vi "BuildRelease.vi"() -> ()   [LabVIEW 2020]
uses:
  <vilib>/Utility/traverseref.llb/TRef TravTarget.ctl
  <vilib>/Utility/traverseref.llb/VI Scripting - Traverse.lvlib
panel:
  out "error out":errorcluster
  out "Tab":enum32{"Start", "Building"}(tab)
  in  "Package Build":i32
  in  "AutoInstallAfterBuild":bool
  in  "DeleteRelease":bool
  in  "Output Folder":path=path "C:/OpenGDS" caption="Build folder: C:\\OpenGDS\\1.2.87(Master)"
  in  "LV_Versions":cluster{"LvVersion":string, "Check":bool}[](array[cluster]) caption="LV versions to compile the release for"
  in  "Build":bool
  out "Branch Name":string
  in  "New Version Number":string
  out "Current Version Number":string
  out "Progress":u8(slide) scale=0.0..100.0
  out "Progress":string
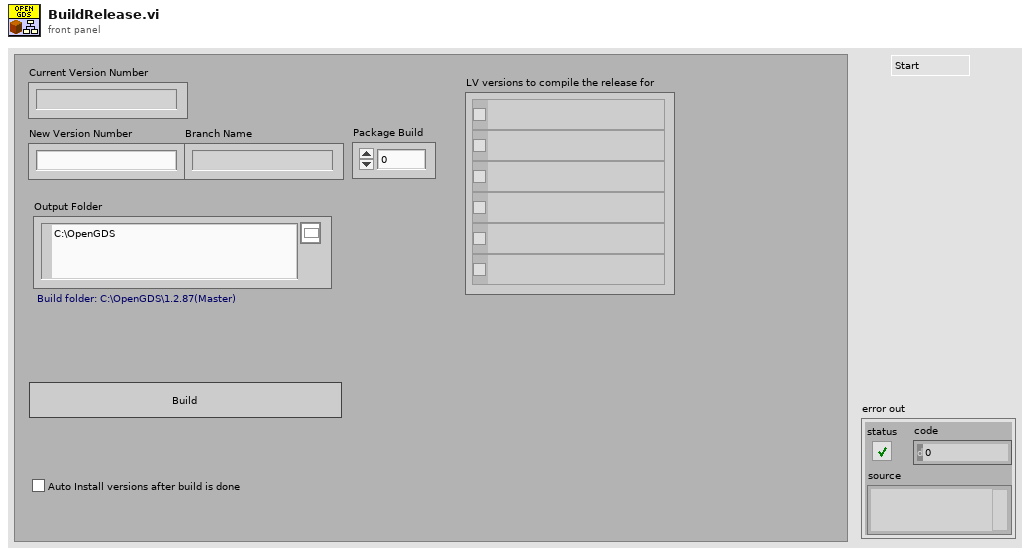
[diagram p1: front panel]
types:
  T1 = cluster{"LvVersion":path[], "BuildPath":path, "SourceFiles":path[], "LvVersion":string[], "SpecFile":path, "IniFiles":path[], "InstallerCopy":path, "VersionName":string, "InstallerFile":path, "ReadMeFile":path, "VIP-File":path, "LogFolder":path, "ZipFilesCreated":path[]}
  T2 = enum32{"invalid OS target", "Mac OS", "Windows 3.1", "Windows 95/NT", "Solaris 1", "Solaris 2", "HP-UX", "PowerMAX", "Linux", "Irix", "Rhapsody", "BeOS", "AIX", "OSF1", "VxWorks", "PharLap", "Carbon", "RTX", "Windows x64", "Linux x64"}
  T3 = enum8{"Enabled", "Disabled", "Disabled and Grayed Out"}
  T4 = typedef "TRef TravTarget.ctl" = enum16{"FP", "BD", "Other"}
  T5 = enum32{"invalid OS target", "Mac OS", "Windows 3.1", "Windows 95/NT", "Solaris 1", "Solaris 2", "HP-UX", "PowerMAX", "Linux", "Irix", "Rhapsody", "BeOS", "AIX", "OSF1", "VxWorks", "PharLap", "Carbon", "RTX", "Windows x64", "Linux x64", "Mac OS X x64"}
  T6 = enum32{"not a typedef", "typedef", "strict typedef", "class private data"}
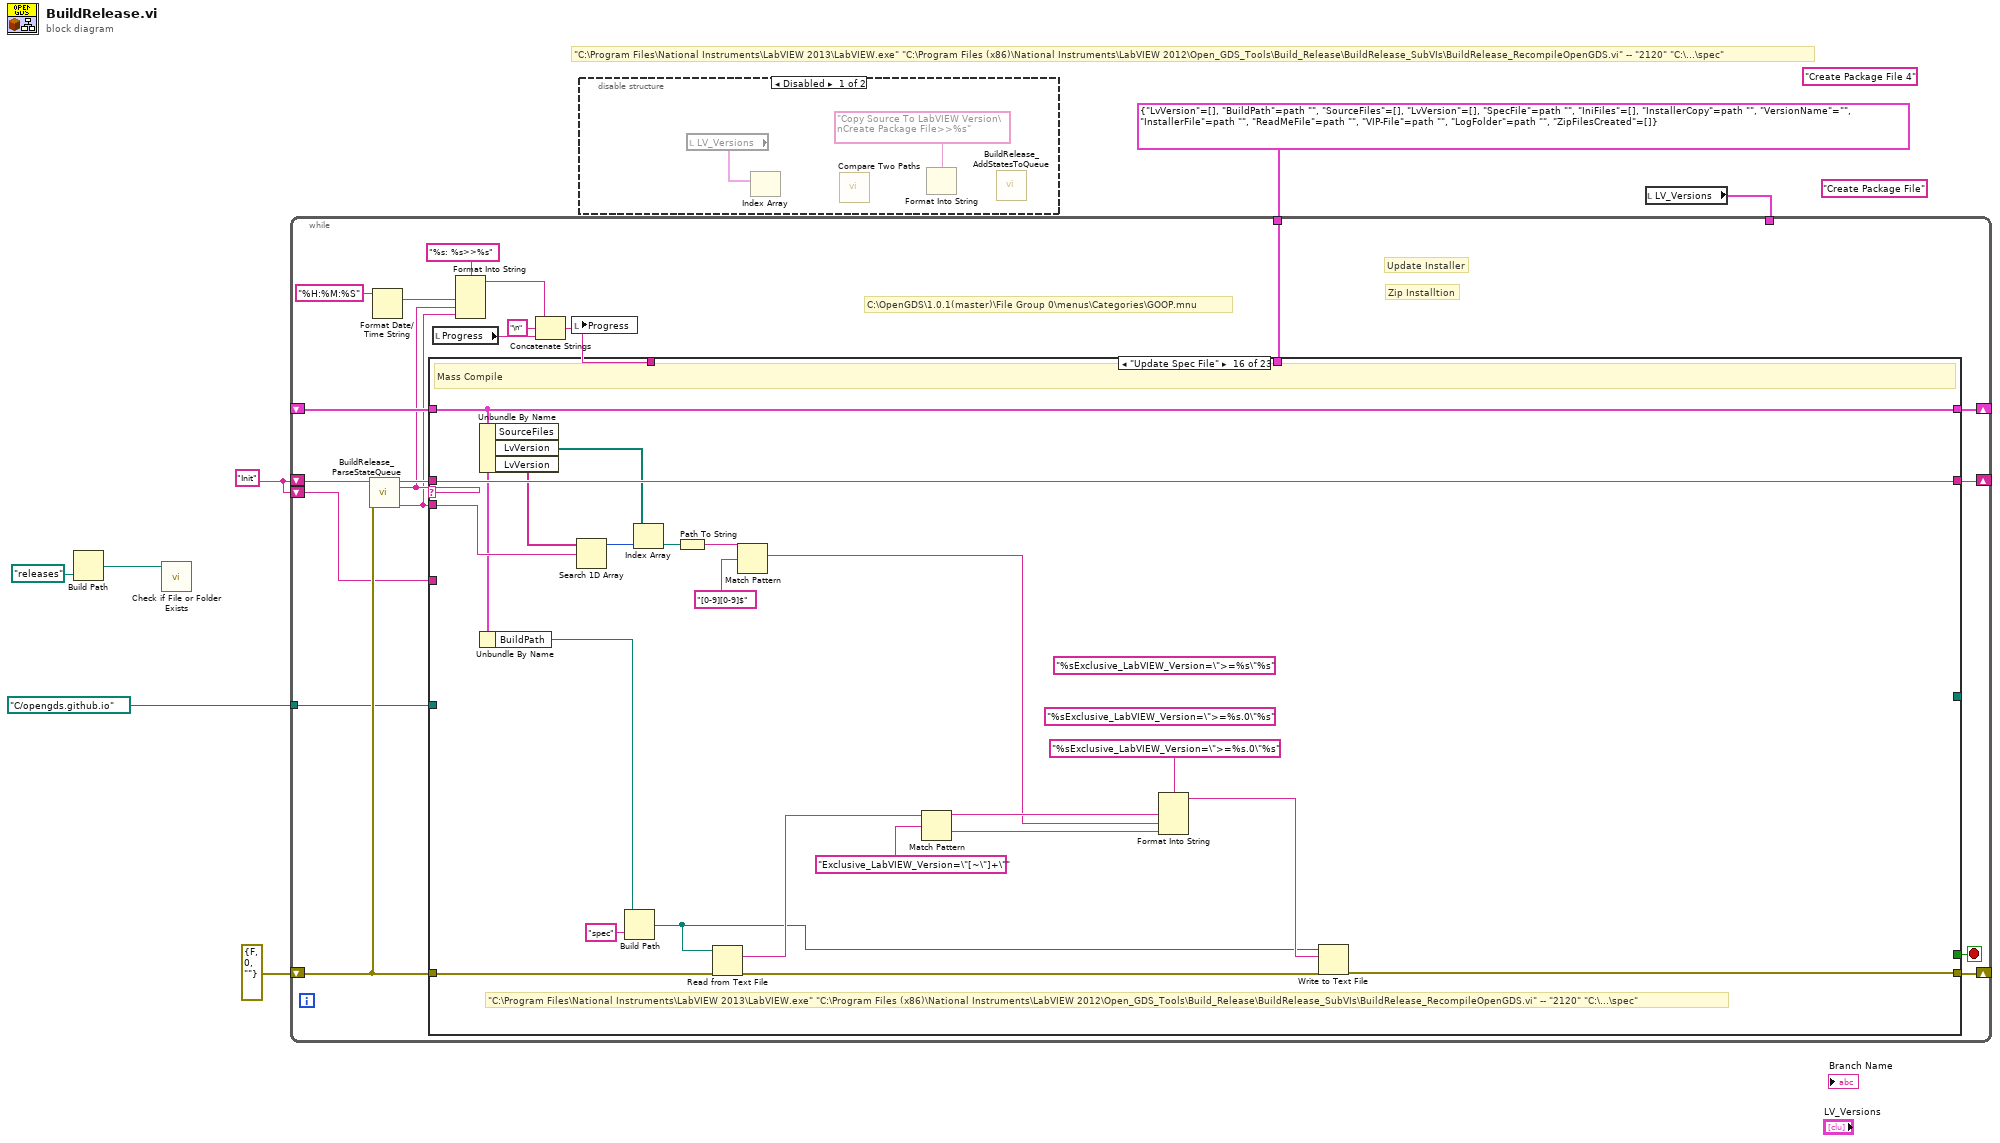
[diagram p0: block diagram]
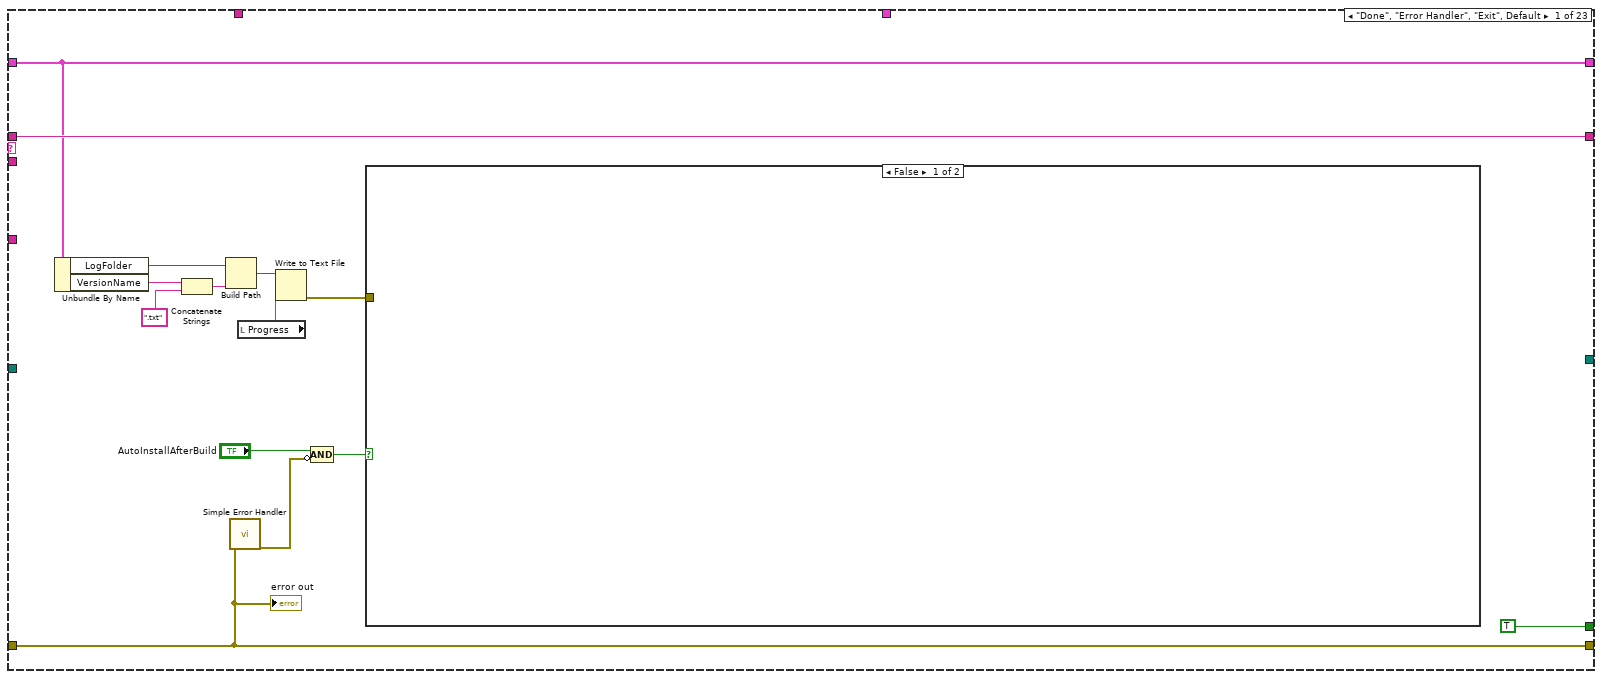
[diagram p3: hidden frame]
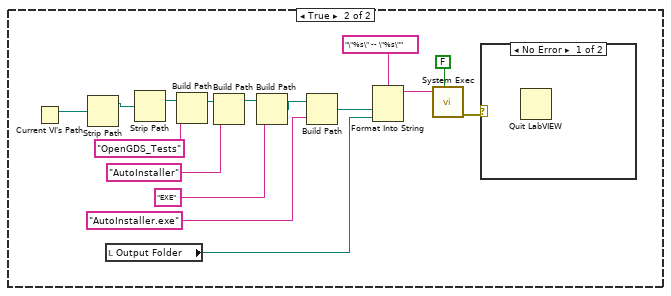
[diagram p4: hidden frame]
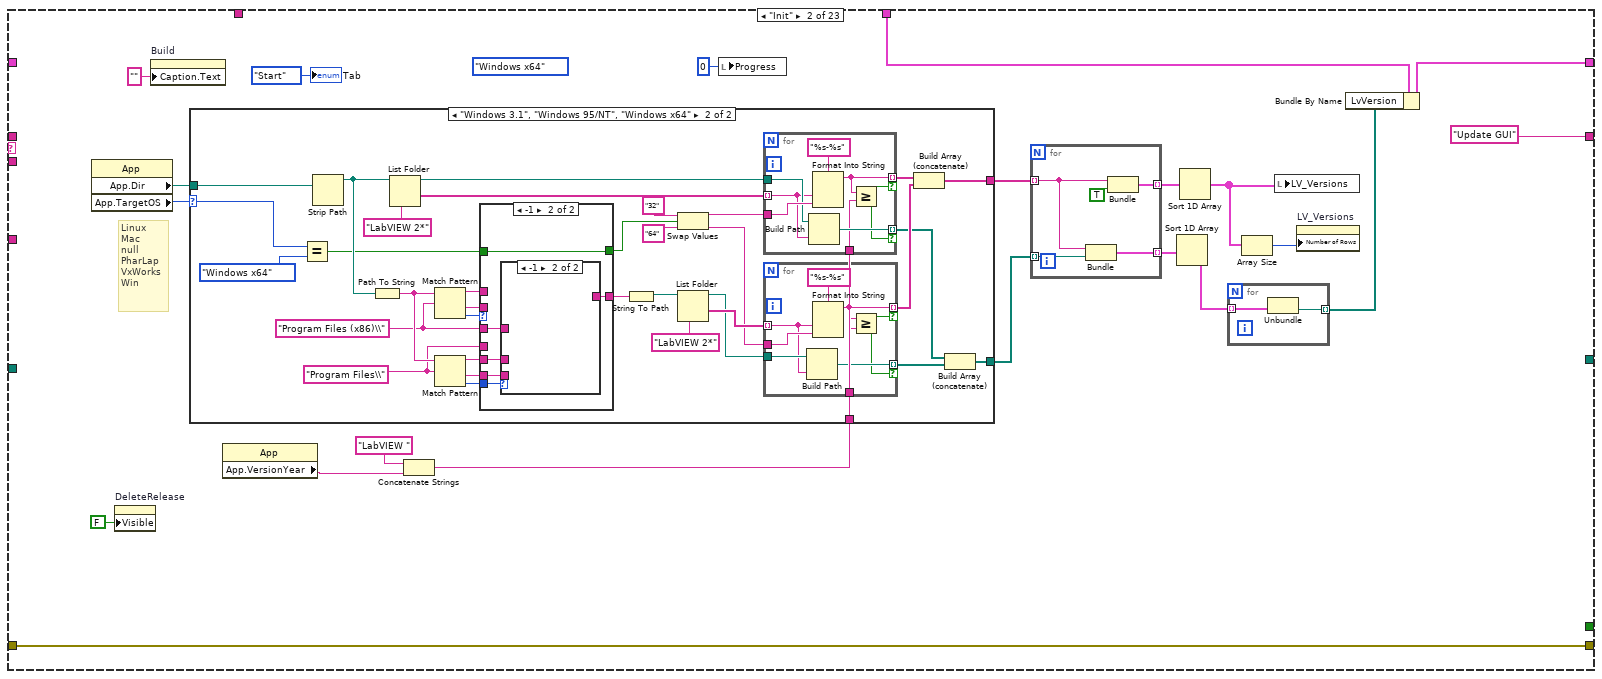
[diagram p6: hidden frame]
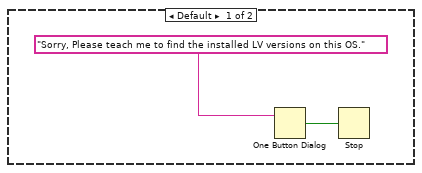
[diagram p7: hidden frame]
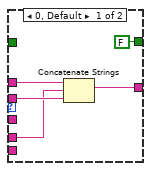
[diagram p8: hidden frame]
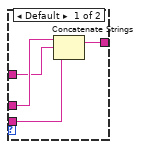
[diagram p9: hidden frame]
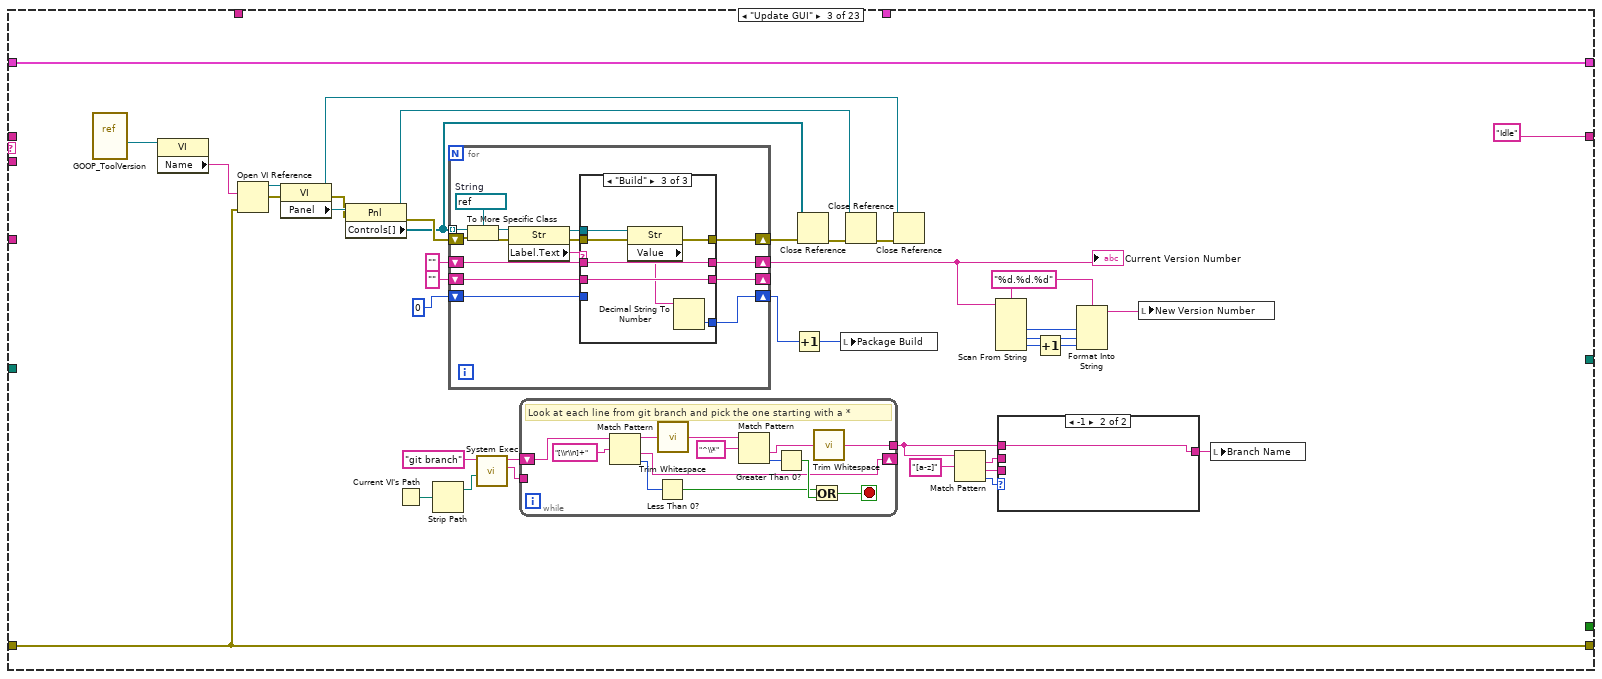
[diagram p10: hidden frame]
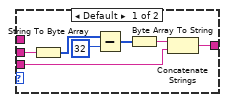
[diagram p11: hidden frame]
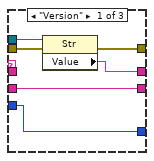
[diagram p12: hidden frame]
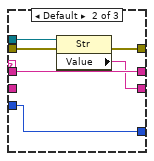
[diagram p13: hidden frame]
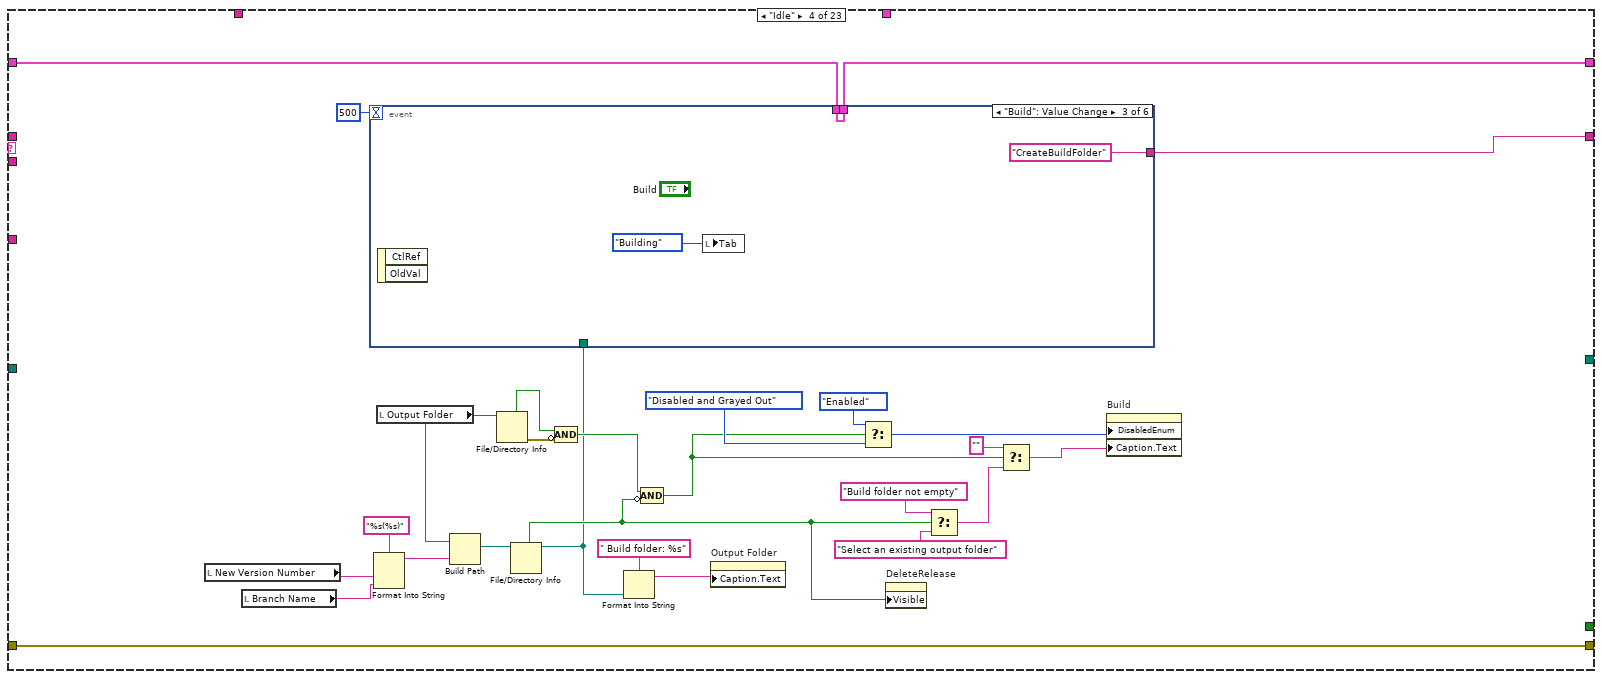
[diagram p14: hidden frame]
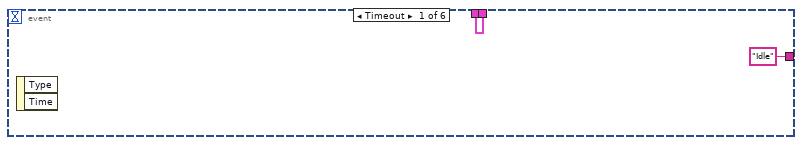
[diagram p15: hidden frame]
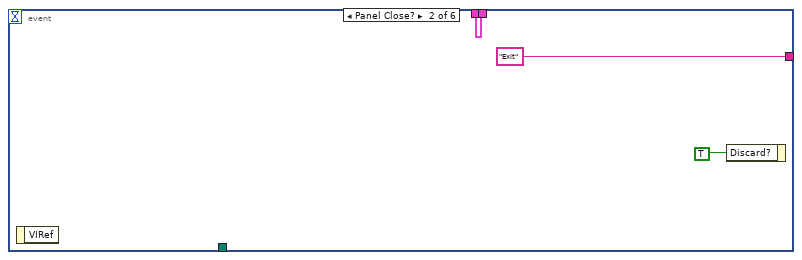
[diagram p16: hidden frame]
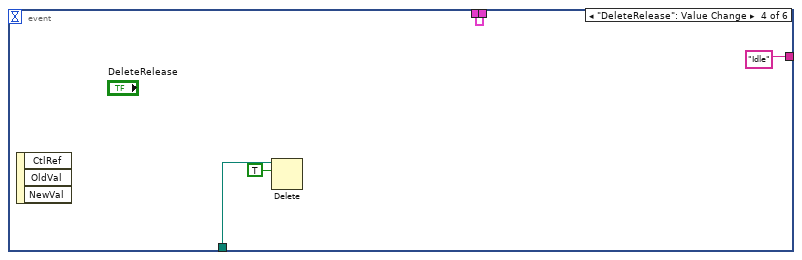
[diagram p17: hidden frame]
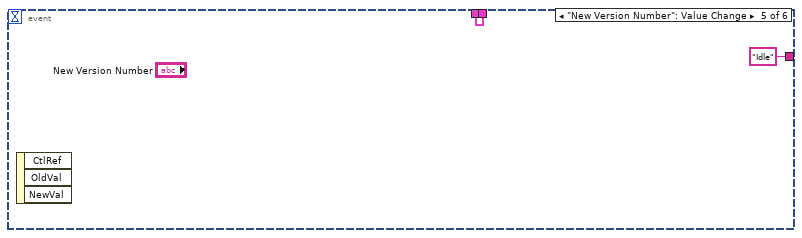
[diagram p18: hidden frame]
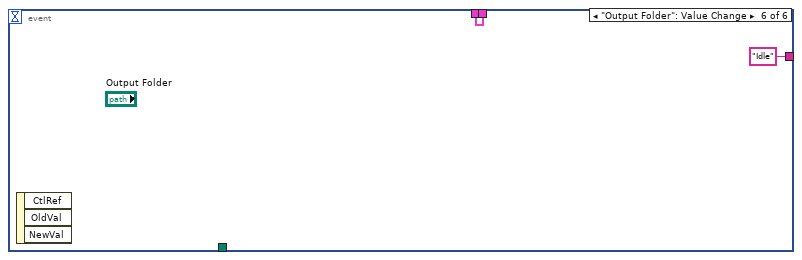
[diagram p19: hidden frame]
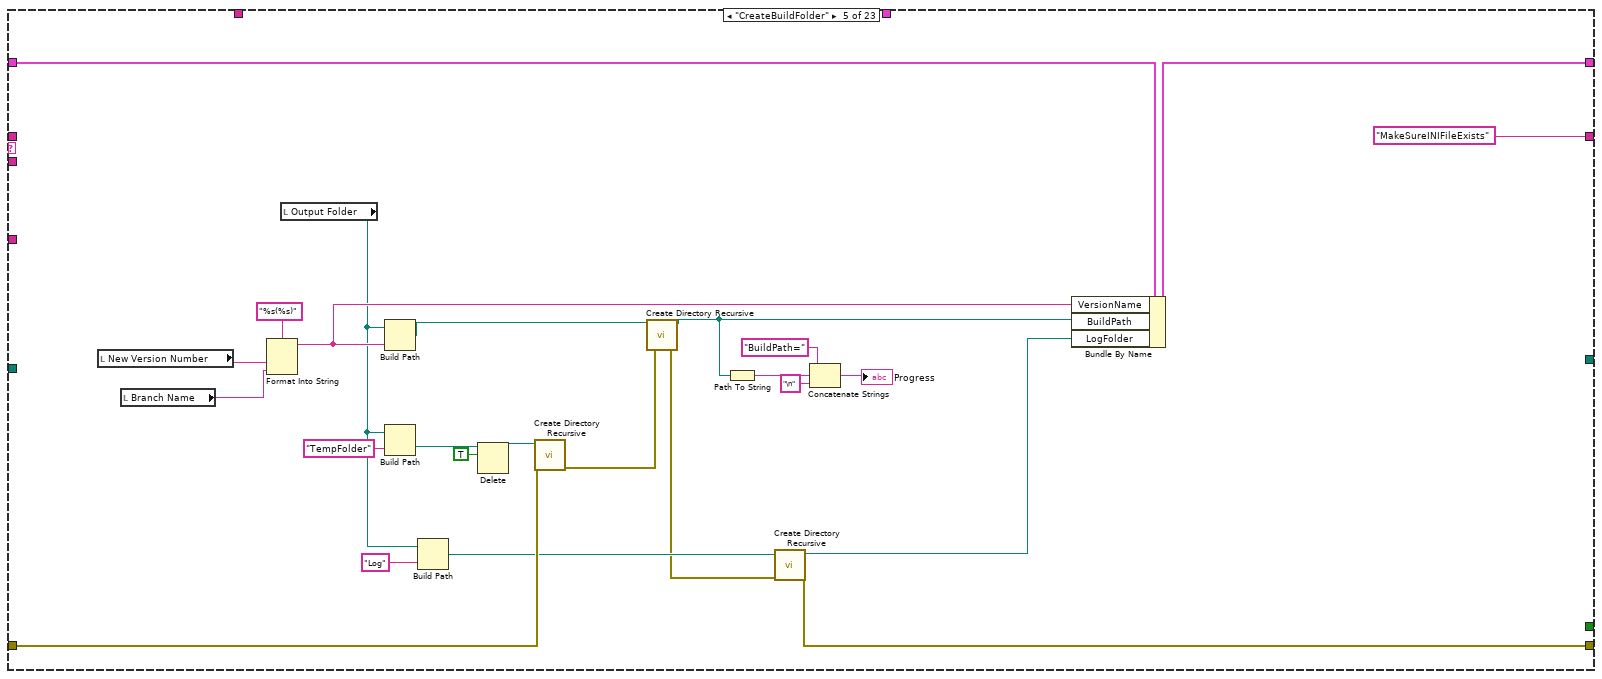
[diagram p20: hidden frame]
diagram:
  (unwired) "Create Package File 4"
  (unwired) "Create Package File"
  w4 = "Init"
  # "\"C:\\Program Files\\National Instruments\\LabVIEW 2013\\LabVIEW.exe\" \"C:\\Program Files (x86)\\National Instruments\\LabVIEW 2012\\Open_GDS_Tools\\Build_Release\\BuildRelease_SubVIs\\BuildRelease_RecompileOpenGDS.vi\" -- \"2120\" \"C:\\...\\spec\""
  n1 = Build Path(name or relative path=path "releases") -> (appended path=w2:path)  [unwired: 1 in]
  n2 = call <vilib>:"Check if File or Folder Exists.vi"("path"=w2) -> ()  [unwired: 8 in, 3 out]
  n3 = disable-structure shown="Disabled" {
    frame Disabled {
      n4 = local read "LV_Versions"() -> (w8:cluster{"LvVersion":string, "Check":bool}[])
      n5 = Index Array(array=w8) -> ()  [unwired: 1 in, 1 out]
      n6 = call <vilib>:"Compare Two Paths.vi"() -> ()  [unwired: 8 in, 4 out]
      n7 = Format Into String(format string="Copy Source To LabVIEW Version\nCreate Package File>>%s") -> ()  [unwired: 3 in, 2 out]
      n8 = call "BuildRelease_AddStatesToQueue.vi"() -> ()  [unwired: 15 in, 1 out]
    }
    frame Enabled {
    }
  }
  n9 = local read "LV_Versions"() -> (w5:cluster{"LvVersion":string, "Check":bool}[])
  n10 = while {
    shift-right: [w29] -> _
    shift-left: errorcluster {"status"=FALSE, "code"=0, "source"=""} ("error IO") -> [w23]
    shift-right: [w22] -> _
    shift-left: w4 -> [w25]
    shift-right: [w28] -> _
    shift-left: _ -> [w27]
    tunnel: T1 {"LvVersion"=[], "BuildPath"=path "", "SourceFiles"=[], "LvVersion"=[], "SpecFile"=path "", "IniFiles"=[], "InstallerCopy"=path "", "VersionName"="", "InstallerFile"=path "", "ReadMeFile"=path "", "VIP-File"=path "", "LogFolder"=path "", "ZipFilesCreated"=[]} -> [w26]
    tunnel: w5 -> [_]
    shift-left: w4 -> [w11]
    tunnel: path "C:/opengds.github.io" -> [w10]
    stop <- w21 stop-if-true
    # "Zip Installtion"
    # "Update Installer"
    # "C:\\OpenGDS\\1.0.1(master)\\File Group 0\\menus\\Categories\\GOOP.mnu"
    n11 = call "BuildRelease_ParseStateQueue.vi"("State Queue"=w25, "Error In (no error)"=w23) -> ("Remaining States"=w24:string, "Current State"=w17:string, "Arguments"=w16:string)  [unwired: 11 in]
    n12 = Format Date/Time String(time format string (%c)="%H:%M:%S") -> (date/time string=w12:string)  [unwired: 2 in]
    n13 = local read "Progress"() -> (w19:string)
    n14 = Format Into String(format string="%s: %s>>%s", w12, w17, w16) -> (resulting string=w15:string)  [unwired: 2 in, 1 out]
    n15 = Concatenate Strings(w15, "\n" ("string"), w19) -> (w18:string)
    n16 = case shown="\"Update Spec File\"" w17 {
      tunnel: w23 -> [w30 w80 w176 w273 w301 w318 w358 w413 w494 w505 w564 w617 w638 w680 w735 w824 w842 w895 w917 w936 w976 w990 w1017]
      tunnel: [w30 w80 w176 w273 w293 w317 w345 w401 w487 w504 w565 w617 w638 w664 w762 w809 w841 w883 w916 w942 w976 w990 w1017] -> w29
      tunnel: [w41 w79 w193 w274 w312 w331 w344 w397 w496 w508 w563 w607 w637 w663 w761 w825 w832 w878 w919 w932 w975 w983 w1010] -> w28
      tunnel: w27 -> [w41 _ w193 w275 w316 w331 w344 w416 w496 w508 w588 w615 w637 w686 w770 w825 w832 w896 w924 w929 w975 w983 w1010]
      tunnel: w26 -> [_ w78 _ _ _ _ _ _ _ _ _ _ _ _ _ _ _ _ _ _ _ _ _]
      tunnel: w24 -> [w43 _ _ _ _ _ _ _ _ _ _ _ w636 w685 w782 w830 w840 w894 w923 w950 w974 w989 w1016]
      tunnel: [w43 "Update GUI" "Idle" w251 "MakeSureINIFileExists" "Update Version Global VI" "Create Package File Spec File" "Add Package Extra Files" "Copy Source To LabVIEW Versions" "Copy Installer VI to Build Folder" "Create Build Process" w611 w636 w685 w782 w830 w840 w894 w923 w950 w974 w989 w1016] -> w22
      tunnel: [TRUE _ _ _ _ _ _ _ _ _ _ _ _ _ _ _ _ _ _ _ _ _ _] -> w21
      tunnel: w16 -> [_ _ _ _ _ _ _ _ _ _ _ _ _ w639 w780 w828 w836 w885 w912 w944 _ _ _]
      tunnel: w18 -> [_ _ _ _ _ _ _ _ _ _ _ _ _ _ _ _ _ _ _ _ _ _ _]
      tunnel: w11 -> [_ _ _ _ _ _ _ _ _ _ _ _ _ _ _ _ _ _ _ _ _ _ _]
      tunnel: [_ _ _ _ _ _ _ _ _ _ _ _ _ _ _ _ w831 _ _ _ _ _ _] -> _
      tunnel: w10 -> [_ _ _ _ _ _ _ _ _ _ _ _ _ _ _ _ _ _ _ w928 _ w988 w1012]
      frame "Done", "Error Handler", "Exit", Default {
        n17 = Unbundle By Name(w41) -> ("LogFolder"=w40:path, "VersionName"=w37:string)
        n18 = Concatenate Strings(w37, ".txt" ("format string")) -> (w36:string)
        n19 = Build Path(base path=w40, name or relative path=w36) -> (appended path=w39:path)
        n20 = call <vilib>:"Simple Error Handler.vi"("error in (no error)"=w30) -> ("error out"=w32:errorcluster)  [unwired: 4 in, 4 out]
        n21 = local read "Progress"() -> (w38:string)
        n22 = Write to Text File(file (use dialog)=w39, text=w38) -> (error out=w31:errorcluster)  [unwired: 2 in, 2 out]
        n23 = Compound Arithmetic op=AND("AutoInstallAfterBuild", invert w32) -> (w33:bool)
        n24 = case shown="False" w33 {
          tunnel: w31 -> [_ _]
          frame False {
          }
          frame True {
            n25 = Current VI's Path() -> (path=w57:path)
            n26 = Strip Path(path=w57) -> (stripped path=w56:path)  [unwired: 1 out]
            n27 = local read "Output Folder"() -> (w46:path)
            n28 = Strip Path(path=w56) -> (stripped path=w55:path)  [unwired: 1 out]
            n29 = Build Path(base path=w55, name or relative path="OpenGDS_Tests") -> (appended path=w53:path)
            n30 = Build Path(base path=w53, name or relative path="AutoInstaller") -> (appended path=w51:path)
            n31 = Build Path(base path=w51, name or relative path="EXE") -> (appended path=w49:path)
            n32 = Build Path(base path=w49, name or relative path="AutoInstaller.exe") -> (appended path=w47:path)
            n33 = Format Into String(format string="\"%s\" -- \"%s\"", w47, w46) -> (resulting string=w58:string)  [unwired: 2 in, 1 out]
            n34 = call <vilib>:"System Exec.vi"("wait until completion? (T)"=FALSE, "command line"=w58) -> ("error out"=w44:errorcluster)  [unwired: 6 in, 3 out]
            n35 = case shown="No Error" w44 {
              frame No Error {
                n36 = Quit LabVIEW() -> ()  [unwired: 1 in]
              }
              frame Error {
              }
            }
          }
        }
        "error out" <- w30
      }
      frame "Init" {
        (unwired) T2."Windows x64" ("y")
        # "Linux\nMac\nnull\nPharLap\nVxWorks\nWin"
        n37 = property class="App"() -> ("App.Dir"=w71:path, "App.TargetOS"=w72:T5)  [unwired: 2 in, 2 out]
        n38 = property on="DeleteRelease" class="Bool"("Visible"=FALSE) -> ()  [unwired: 2 in, 2 out]
        n39 = property on="Build" class="Bool"("Caption.Text"="") -> ()  [unwired: 2 in, 2 out]
        n40 = property class="App"() -> ("App.VersionYear"=w69:string)  [unwired: 2 in, 2 out]
        n41 = Concatenate Strings("LabVIEW " ("pattern"), w69) -> (w68:string)
        n42 = case shown="\"Windows 3.1\", \"Windows 95/NT\", \"Windows x64\"" w72 {
          selector: w72 -> [_ w86]
          tunnel: [_ w118] -> w77
          tunnel: w68 -> [_ w117]
          tunnel: [_ w116] -> w64
          tunnel: w71 -> [_ w85]
          frame Default {
            n43 = One Button Dialog(message="Sorry, Please teach me to find the installed LV versions on this OS.") -> (true=w83:bool)  [unwired: 1 in]
            n44 = Stop(stop? (T)=w83) -> ()
          }
          frame "Windows 3.1", "Windows 95/NT", "Windows x64" {
            w109 = "Program Files\\" ("regular expression")
            w94 = "Program Files (x86)\\" ("regular expression")
            n45 = Equal?(x=w86, y=T2."Windows x64") -> (x = y?=w97:bool)
            n46 = Strip Path(path=w85) -> (stripped path=w112:path)  [unwired: 1 out]
            n47 = Path To String(path=w112) -> (string=w114:string)
            n48 = List Folder(path=w112, pattern="LabVIEW 2*") -> (path out=w88:path, folder names=w105:string[])  [unwired: 2 in, 2 out]
            n49 = Match Pattern(string=w114, regular expression=w94) -> (before substring=w111:string, after substring=w110:string, offset past match=w113:i32)  [unwired: 1 in, 1 out]
            n50 = Match Pattern(string=w114, regular expression=w109) -> (before substring=w96:string, after substring=w95:string, offset past match=w99:i32)  [unwired: 1 in, 1 out]
            n51 = case shown="-1" w113 {
              tunnel: w111 -> [w139 _]
              tunnel: w110 -> [w138 _]
              tunnel: w109 -> [w137 _]
              tunnel: [w136 w140] -> w108
              tunnel: [FALSE w144] -> w104
              tunnel: w99 -> [_ w145]
              tunnel: w97 -> [_ w144]
              tunnel: w96 -> [_ w143]
              tunnel: w95 -> [_ w142]
              tunnel: w94 -> [_ w141]
              frame 0, Default {
                n52 = Concatenate Strings(w139, w137, w138) -> (w136:string)
              }
              frame -1 {
                n53 = case shown="-1" w145 {
                  tunnel: w143 -> [w149 _]
                  tunnel: w142 -> [w148 _]
                  tunnel: w141 -> [w147 _]
                  tunnel: [w146 _] -> w140
                  frame Default {
                    n54 = Concatenate Strings(w149, w147, w148) -> (w146:string)
                  }
                  frame -1 {
                  }
                }
              }
            }
            n55 = String To Path(string=w108) -> (path=w106:path)
            n56 = Swap Values(12:"32" ("format string"), 13:w104, 14:"64" ("format string")) -> (1:w101:string, 3:w91:string)
            n57 = List Folder(path=w106, pattern="LabVIEW 2*") -> (path out=w90:path, folder names=w100:string[])  [unwired: 2 in, 2 out]
            n58 = for {
              tunnel: w105 -> [w131] mode=indexing
              tunnel: w101 -> [w133]
              tunnel: [w129] -> w93 mode=indexing if=w127
              tunnel: w88 -> [w132]
              tunnel: [w130] -> w87 mode=indexing if=w127
              tunnel: w117 -> [w128]
              n59 = Build Path(base path=w132, name or relative path=w131) -> (appended path=w130:path)
              n60 = Format Into String(format string="%s-%s", w131, w133) -> (resulting string=w129:string)  [unwired: 2 in, 1 out]
              n61 = Greater Or Equal?(x=w129, y=w128) -> (x >= y?=w127:bool)
            }
            n62 = for {
              tunnel: w100 -> [w123] mode=indexing
              tunnel: w91 -> [w125]
              tunnel: [w121] -> w92 mode=indexing if=w119
              tunnel: w90 -> [w124]
              tunnel: [w122] -> w89 mode=indexing if=w119
              tunnel: w117 -> [w120]
              n63 = Build Path(base path=w124, name or relative path=w123) -> (appended path=w122:path)
              n64 = Format Into String(format string="%s-%s", w123, w125) -> (resulting string=w121:string)  [unwired: 2 in, 1 out]
              n65 = Greater Or Equal?(x=w121, y=w120) -> (x >= y?=w119:bool)
            }
            n66 = Build Array (concatenate)(w93, w92) -> (w118:string[])
            n67 = Build Array (concatenate)(w87, w89) -> (w116:path[])
          }
        }
        n68 = local write "Progress"(u8 0 ("Progress")) -> ()
        n69 = for {
          tunnel: w77 -> [w153] mode=indexing
          tunnel: [w154] -> w76 mode=indexing
          tunnel: w64 -> [w152] mode=indexing
          tunnel: [w151] -> w62 mode=indexing
          n70 = Bundle(w153, "appended path"=w152) -> (w151:cluster{string, "appended path":path})  [unwired: 1 in]
          n71 = Bundle(w153, "Check"=TRUE) -> (w154:cluster{string, "Check":bool})  [unwired: 1 in]
        }
        n72 = Sort 1D Array(array=w62) -> (sorted array=w61:cluster{string, "appended path":path}[])
        n73 = Sort 1D Array(array=w76) -> (sorted array=w63:cluster{string, "Check":bool}[])
        n74 = for {
          tunnel: w61 -> [w82] mode=indexing
          tunnel: [w81] -> w60 mode=indexing
          n75 = Unbundle(w82) -> ("appended path"=w81:path)  [unwired: 1 out]
        }
        n76 = Array Size(array=w63) -> (size(s)=w75:i32)
        n77 = local write "LV_Versions"(w63) -> ()
        n78 = property on="LV_Versions" class="Arr (strict)"("Number of Rows"=w75) -> ()  [unwired: 2 in, 2 out]
        n79 = Bundle By Name(cluster=w78, "LvVersion"=w60) -> (w79:T1)
        "Tab" <- enum32{"Start", "Building"}."Start" ("Tab")
      }
      frame "Update GUI" {
        w192 = "%d.%d.%d" ("format string")
        n80 = vi-ref "GOOP_ToolVersion.vi"() -> (w183:refnum<vi>)
        n81 = property class="VI"(reference=w183) -> ("Name"=w182:string)  [unwired: 1 in, 2 out]
        n82 = Open VI Reference(vi path=w182, error in (no error)=w176) -> (vi reference=w181:refnum<vi>, error out=w180:errorcluster)  [unwired: 4 in]
        n83 = property class="VI"(reference=w181, error in=w180) -> (reference out=w170:refnum<vi>, error out=w177:errorcluster, "Panel"=w179:refnum<vi>)
        n84 = property class="Pnl"(reference=w179, error in=w177) -> (reference out=w172:refnum<vi>, error out=w178:errorcluster, "Controls[]"=w174:refnum<vi>[])
        n85 = Current VI's Path() -> (path=w186:path)
        n86 = Strip Path(path=w186) -> (stripped path=w185:path)  [unwired: 1 out]
        n87 = for {
          tunnel: w174 -> [w228] mode=indexing
          shift-right: [w224] -> w175
          shift-left: w178 -> [w221]
          shift-right: [w220] -> w167
          shift-left: "" ("Value") -> [w219]
          shift-right: [w218] -> _
          shift-left: "" ("Value") -> [w217]
          shift-right: [w215] -> w156
          shift-left: 0 -> [w216]
          w227 = refnum<vi> refnum  # String
          n88 = To More Specific Class(target class=w227, reference=w228, error in=w221) -> (specific class reference=w226:refnum<vi>, error out=w222:errorcluster)
          n89 = property class="Str"(reference=w226, error in=w222) -> (reference out=w225:refnum<vi>, error out=w223:errorcluster, "Label.Text"=w229:string)
          n90 = case shown="\"Build\"" w229 {
            tunnel: w225 -> [w235 w241 w248]
            tunnel: [w233 w240 w247] -> w224
            tunnel: w223 -> [w234 w239 w246]
            tunnel: [w232 w238 w245] -> w220
            tunnel: w219 -> [_ w238 w245]
            tunnel: [w231 w237 w244] -> w218
            tunnel: w217 -> [w231 _ w244]
            tunnel: w216 -> [w230 w236 _]
            tunnel: [w230 w236 w242] -> w215
            frame "Version" {
              n91 = property class="Str"(reference=w235, error in=w234) -> (error out=w233:errorcluster, "Value"=w232:string)  [unwired: 1 out]
            }
            frame Default {
              n92 = property class="Str"(reference=w241, error in=w239) -> (error out=w240:errorcluster, "Value"=w237:string)  [unwired: 1 out]
            }
            frame "Build" {
              n93 = property class="Str"(reference=w248, error in=w246) -> (error out=w247:errorcluster, "Value"=w243:string)  [unwired: 1 out]
              n94 = Decimal String To Number(string=w243) -> (number=w242:i32)  [unwired: 2 in, 1 out]
            }
          }
        }
        "Current Version Number" <- w167
        n95 = call <vilib>:"System Exec.vi"("working directory"=w185, "command line"="git branch") -> ("standard error"=w158:string, "standard output"=w159:string)  [unwired: 6 in, 2 out]
        n96 = while {
          tunnel: [w194] -> w160
          shift-right: [w197] -> _
          shift-left: w159 -> [w201]
          tunnel: w158 -> [_]
          stop <- w200 stop-if-true
          # "Look at each line from git branch and pick the one starting with a *"
          n97 = Match Pattern(string=w201, regular expression="[\\r\\n]+") -> (before substring=w198:string, after substring=w197:string, offset past match=w199:i32)  [unwired: 1 in, 1 out]
          n98 = Less Than 0?(x=w199) -> (x < 0?=w195:bool)
          n99 = call <vilib>:"Trim Whitespace.vi"("string"=w198) -> ("trimmed string"=w206:string)  [unwired: 1 in]
          n100 = Match Pattern(string=w206, regular expression="^\\*") -> (after substring=w204:string, offset past match=w203:i32)  [unwired: 1 in, 2 out]
          n101 = Greater Than 0?(x=w203) -> (x > 0?=w202:bool)
          n102 = Or(x=w195, y=w202) -> (x .or. y?=w200:bool)
          n103 = call <vilib>:"Trim Whitespace.vi"("string"=w204) -> ("trimmed string"=w194:string)  [unwired: 1 in]
        }
        n104 = Increment(x=w156) -> (x+1=w155:i32)
        n105 = Close Reference(reference=w174, error in (no error)=w175) -> (error out=w173:errorcluster)
        n106 = local write "Package Build"(w155) -> ()
        n107 = Close Reference(reference=w172, error in (no error)=w173) -> (error out=w171:errorcluster)
        n108 = Close Reference(reference=w170, error in (no error)=w171) -> ()  [unwired: 1 out]
        n109 = Match Pattern(string=w160, regular expression="[a-z]") -> (match substring=w162:string, after substring=w161:string, offset past match=w164:i32)  [unwired: 1 in, 1 out]
        n110 = Scan From String(format string=w192, input string=w167) -> (output 1=w191:i32, output 2=w190:i32, output 3=w189:i32)  [unwired: 5 in, 3 out]
        n111 = case shown="-1" w164 {
          tunnel: w160 -> [_ w214]
          tunnel: [w207 w214] -> w163
          tunnel: w162 -> [w213 _]
          tunnel: w161 -> [w208 _]
          frame Default {
            n112 = String To Byte Array(string=w213) -> (unsigned byte array=w212:u8[])
            n113 = Subtract(x=w212, y=32) -> (x-y=w210:i32[])
            n114 = Byte Array To String(unsigned byte array=w210) -> (string=w209:string)
            n115 = Concatenate Strings(w209, w208) -> (w207:string)
          }
          frame -1 {
          }
        }
        n116 = Increment(x=w189) -> (x+1=w188:i32)
        n117 = Format Into String(format string=w192, w191, w190, w188) -> (resulting string=w187:string)  [unwired: 2 in, 1 out]
        n118 = local write "New Version Number"(w187) -> ()
        n119 = local write "Branch Name"(w163) -> ()
      }
      frame "Idle" {
        n120 = local read "New Version Number"() -> (w264:string)
        n121 = local read "Branch Name"() -> (w265:string)
        n122 = Format Into String(format string="%s(%s)", w264, w265) -> (resulting string=w262:string)  [unwired: 2 in, 1 out]
        n123 = local read "Output Folder"() -> (w260:path)
        n124 = Build Path(base path=w260, name or relative path=w262) -> (appended path=w261:path)
        n125 = File/Directory Info(path=w260) -> (directory=w271:bool, error out=w272:errorcluster)  [unwired: 1 in, 5 out]
        n126 = File/Directory Info(path=w261) -> (path out=w249:path, directory=w250:bool)  [unwired: 1 in, 5 out]
        n127 = event shown="[2] \"Build\": Value Change" {
          selector: _ -> [_ _ _ _ _ _]
          dyn-events: _ -> [_ _ _ _ _ _]
          timeout: 500 -> [_ _ _ _ _ _]
          tunnel: w275 -> [w277 w279 w283 w287 w289 w291]
          tunnel: [w277 w279 w283 w287 w289 w291] -> w274
          tunnel: ["Idle" "Exit" "CreateBuildFolder" "Idle" "Idle" "Idle"] -> w251
          tunnel: w249 -> [_ _ _ w286 _ _]
          event Timeout {
            n128 = event-data() -> ()  [unwired: 1 in, 2 out]
          }
          event Panel Close? {
            n129 = event-data() -> ()  [unwired: 1 in, 1 out]
            n130 = event-data("Discard?"=TRUE) -> ()  [unwired: 1 in, 1 out]
          }
          event "Build": Value Change {
            n131 = event-data() -> ()  [unwired: 1 in, 2 out]
            n132 = local write "Tab"(enum32{"Start", "Building"}."Building" ("Tab")) -> ()
          }
          event "DeleteRelease": Value Change {
            n133 = event-data() -> ()  [unwired: 1 in, 3 out]
            n134 = Delete(path (use dialog)=w286, entire hierarchy (F)=TRUE) -> ()  [unwired: 3 in, 3 out]
          }
          event "New Version Number": Value Change {
            n135 = event-data() -> ()  [unwired: 1 in, 3 out]
          }
          event "Output Folder": Value Change {
            n136 = event-data() -> ()  [unwired: 1 in, 3 out]
          }
        }
        n137 = Compound Arithmetic op=AND(w271, invert w272) -> (w258:bool)
        n138 = Format Into String(format string=" Build folder: %s", w249) -> (resulting string=w253:string)  [unwired: 2 in, 1 out]
        n139 = Compound Arithmetic op=AND(w258, invert w250) -> (w259:bool)
        n140 = property on="Output Folder" class="Path"("Caption.Text"=w253) -> ()  [unwired: 2 in, 2 out]
        n141 = Select(t=T3."Enabled" ("Disabled"), s=w259, f=T3."Disabled and Grayed Out" ("Disabled")) -> (s? t:f=w270:T3)
        n142 = property on="DeleteRelease" class="Bool"("Visible"=w250) -> ()  [unwired: 2 in, 2 out]
        n143 = Select(t="Build folder not empty" ("Caption.Text"), s=w250, f="Select an existing output folder" ("Caption.Text")) -> (s? t:f=w255:string)
        n144 = Select(t="" ("Caption.Text"), s=w259, f=w255) -> (s? t:f=w266:string)
        n145 = property on="Build" class="Bool"("DisabledEnum"=w270, "Caption.Text"=w266) -> ()  [unwired: 2 in, 2 out]
      }
      frame "CreateBuildFolder" {
        n146 = local read "New Version Number"() -> (w314:string)
        n147 = local read "Branch Name"() -> (w315:string)
        n148 = Format Into String(format string="%s(%s)", w314, w315) -> (resulting string=w298:string)  [unwired: 2 in, 1 out]
        n149 = local read "Output Folder"() -> (w297:path)
        n150 = Build Path(base path=w297, name or relative path=w298) -> (appended path=w304:path)
        n151 = Build Path(base path=w297, name or relative path="TempFolder") -> (appended path=w306:path)
        n152 = Build Path(base path=w297, name or relative path="Log") -> (appended path=w295:path)
        n153 = Delete(path (use dialog)=w306, entire hierarchy (F)=TRUE) -> (deleted path=w302:path)  [unwired: 3 in, 2 out]
        n154 = call <vilib>:"Create Directory Recursive.vi"("error in (no error)"=w301, "directory"=w302) -> ("error out"=w300:errorcluster)  [unwired: 3 in, 2 out]
        n155 = call <vilib>:"Create Directory Recursive.vi"("error in (no error)"=w300, "directory"=w304) -> ("error out"=w294:errorcluster, "directory copy"=w303:path)  [unwired: 3 in, 1 out]
        n156 = Path To String(path=w303) -> (string=w310:string)
        n157 = call <vilib>:"Create Directory Recursive.vi"("error in (no error)"=w294, "directory"=w295) -> ("error out"=w293:errorcluster, "directory copy"=w292:path)  [unwired: 3 in, 1 out]
        n158 = Concatenate Strings("BuildPath=" ("string"), w310, "\n" ("string")) -> (→"Progress":string)
        n159 = Bundle By Name(cluster=w316, "VersionName"=w298, "BuildPath"=w303, "LogFolder"=w292) -> (w312:T1)
      }
      frame "MakeSureINIFileExists" {
        # "INI-FILES-GProviders"
        n160 = property class="App"() -> ("App.Dir"=w321:path)  [unwired: 2 in, 2 out]
        n161 = Current VI's Path() -> (path=w329:path)
        n162 = Strip Path(path=w329) -> (stripped path=w328:path)  [unwired: 1 out]
        n163 = Strip Path(path=w328) -> (stripped path=w327:path)  [unwired: 1 out]
        n164 = for {
          shift-right: [w333] -> w319
          shift-left: w321 -> [w334]
          tunnel: string[] ["resource", "Framework", "Providers", "GProviders"] -> [w332] mode=indexing
          n165 = Build Path(base path=w334, name or relative path=w332) -> (appended path=w333:path)
        }
        n166 = Build Path(base path=w327, name or relative path="INI-FILES-GProviders" ("string")) -> (appended path=w325:path)
        n167 = call <vilib>:"Recursive File List.vi"("pattern"="*.ini", "error in (no error)"=w318, "Folder Path"=w325) -> ("error out"=w322:errorcluster, "All Files in Dir"=w323:path[])  [unwired: 4 in, 3 out]
        n168 = for {
          tunnel: w323 -> [w339] mode=indexing
          shift-right: [w335] -> w317
          shift-left: w322 -> [w338]
          tunnel: w319 -> [w336]
          n169 = Copy(8:w338, 9:TRUE ("overwrite (F)"), 10:w336, 11:w339) -> (0:w335:errorcluster)  [unwired: 1 in, 2 out]
        }
      }
      frame "Update Version Global VI" {
        n170 = vi-ref "GOOP_ToolVersion.vi"() -> (w360:refnum<vi>)
        n171 = property class="VI"(reference=w360) -> ("Name"=w359:string)  [unwired: 1 in, 2 out]
        n172 = Open VI Reference(vi path=w359, error in (no error)=w358) -> (vi reference=w357:refnum<vi>, error out=w356:errorcluster)  [unwired: 4 in]
        n173 = property class="VI"(reference=w357, error in=w356) -> (reference out=w346:refnum<vi>, error out=w352:errorcluster, "Panel"=w355:refnum<vi>)
        n174 = property class="Pnl"(reference=w355, error in=w352) -> (error out=w353:errorcluster, "Controls[]"=w354:refnum<vi>[])  [unwired: 1 out]
        n175 = local read "New Version Number"() -> (w342:string)
        n176 = local read "Branch Name"() -> (w343:string)
        n177 = local read "Package Build"() -> (w340:i32)
        n178 = for {
          tunnel: w354 -> [w371] mode=indexing
          shift-right: [w367] -> w347
          shift-left: w353 -> [w364]
          tunnel: w342 -> [w363]
          tunnel: w343 -> [w362]
          tunnel: w340 -> [w361]
          w370 = refnum<vi> refnum  # String
          n179 = To More Specific Class(target class=w370, reference=w371, error in=w364) -> (specific class reference=w369:refnum<vi>, error out=w365:errorcluster)
          n180 = property class="Str"(reference=w369, error in=w365) -> (reference out=w368:refnum<vi>, error out=w366:errorcluster, "Label.Text"=w372:string)
          n181 = case shown="\"Build\"" w372 {
            tunnel: w368 -> [w376 w381 w385]
            tunnel: [w374 w379 w384] -> w367
            tunnel: w366 -> [w375 w380 w383]
            tunnel: w363 -> [w373 _ _]
            tunnel: w362 -> [_ _ w382]
            tunnel: w361 -> [_ w378 _]
            frame "Version" {
              n182 = property class="Str"(reference=w376, error in=w375, "Value"=w373) -> (error out=w374:errorcluster)  [unwired: 1 out]
            }
            frame "Build" {
              n183 = Number To Decimal String(number=w378) -> (decimal integer string=w377:string)  [unwired: 1 in]
              n184 = property class="Str"(reference=w381, error in=w380, "Value"=w377) -> (error out=w379:errorcluster)  [unwired: 1 out]
            }
            frame Default {
              n185 = property class="Str"(reference=w385, error in=w383, "Value"=w382) -> (error out=w384:errorcluster)  [unwired: 1 out]
            }
          }
        }
        n186 = invoke class="VI" method="Default Vals.Make Curr Default"(reference=w346, error in=w347) -> (reference out=w349:refnum<vi>, error out=w348:errorcluster)  [unwired: 1 in, 1 out]
        n187 = invoke class="VI" method="Save.Instrument"(reference=w349, error in=w348) -> (reference out=w350:refnum<vi>, error out=w351:errorcluster)  [unwired: 4 in, 4 out]
        n188 = Close Reference(reference=w350, error in (no error)=w351) -> (error out=w345:errorcluster)
      }
      frame "Create Package File Spec File" {
        # "Create The Spec file"
        n189 = Current VI's Path() -> (path=w434:path)
        n190 = Strip Path(path=w434) -> (stripped path=w420:path)  [unwired: 1 out]
        n191 = Build Path(base path=w420, name or relative path="OpenGDS_FileList.txt") -> (appended path=w430:path)
        n192 = Build Path(base path=w420, name or relative path="vipm-files") -> (appended path=w419:path)
        n193 = property class="App"() -> ("App.Dir"=w431:path)  [unwired: 2 in, 2 out]
        n194 = Read from Text File(file (use dialog)=w430, error in=w413) -> (text=w429:string, error out=w412:errorcluster)  [unwired: 2 in, 2 out]
        n195 = call <vilib>:"Trim Whitespace.vi"("string"=w429) -> ("trimmed string"=w428:string)  [unwired: 1 in]
        n196 = Build Path(base path=w419, name or relative path="vipm_spec_template.txt") -> (appended path=w423:path)
        n197 = Spreadsheet String To Array(delimiter (Tab)="\n", format string="%s", spreadsheet string=w428, array type (2D Dbl)=string[] []) -> (array=w424:string[])
        n198 = Read from Text File(file (use dialog)=w423, error in=w412) -> (text=w392:string, error out=w411:errorcluster)  [unwired: 2 in, 2 out]
        n199 = for {
          tunnel: w431 -> [w455]
          tunnel: w424 -> [w456] mode=indexing
          tunnel: [w450] -> w409 mode=concatenating
          n200 = Build Path(base path=w455, name or relative path=w456) -> (appended path=w454:path)
          n201 = File/Directory Info(path=w454) -> (path out=w451:path, directory=w452:bool, error out=w453:errorcluster)  [unwired: 1 in, 4 out]
          n202 = case shown="No Error" w453 {
            selector: w453 -> [w458 _]
            tunnel: w452 -> [w460 _]
            tunnel: w451 -> [w459 _]
            tunnel: [w457 _] -> w450
            frame No Error {
              n203 = case shown="False" w460 {
                tunnel: w459 -> [w462 w465]
                tunnel: w458 -> [_ w464]
                tunnel: [w461 w463] -> w457
                frame False {
                  n204 = Build Array(w462) -> (w461:path[])
                }
                frame True {
                  n205 = call <vilib>:"Recursive File List.vi"("error in (no error)"=w464, "Folder Path"=w465) -> ("All Files in Dir"=w463:path[])  [unwired: 5 in, 4 out]
                }
              }
            }
            frame Error {
            }
          }
        }
        n206 = local read "New Version Number"() -> (w390:string)
        n207 = Format Into String(format string=".%d", initial string=w390, "Package Build") -> (resulting string=w387:string)  [unwired: 1 in, 1 out]
        n208 = Search and Replace String(input string=w392, search string="<version>", replace string=w387) -> (result string=w393:string)  [unwired: 5 in, 3 out]
        n209 = Array Size(array=w409) -> (size(s)=w395:i32)
        n210 = stacked-sequence {
          tunnel: w395 -> [_]
          tunnel: [w435] -> w394
          frame #0 {
            n211 = Format Date/Time String(time format string (%c)="%H:%M: ") -> (date/time string=w435:string)  [unwired: 2 in]
          }
        }
        n212 = Bundle By Name(cluster=w416, "SourceFiles"=w409) -> (w410:T1)
        n213 = Format Into String(format string="%d\n", initial string=w393, w395) -> (resulting string=w421:string)  [unwired: 1 in, 1 out]
        n214 = Format Into String(format string="Files:%d", initial string=w394, w395) -> (resulting string=w403:string)  [unwired: 1 in, 1 out]
        n215 = local read "Progress"() -> (w406:string)
        n216 = for {
          tunnel: w409 -> [w443] mode=indexing
          shift-right: [w445] -> w398
          shift-left: w421 -> [w449]
          tunnel: [w438] -> w386 mode=indexing if=w437
          i -> [w447]
          n217 = Path To String(path=w443) -> (string=w444:string)
          n218 = Strip Path(path=w443) -> (name=w442:string)  [unwired: 1 out]
          n219 = Match Pattern(string=w444, regular expression="LabVIEW [0-9]+[\\\\/]") -> (after substring=w439:string)  [unwired: 1 in, 3 out]
          n220 = Match Pattern(string=w442, regular expression="^GOOP_[A-Za-z]+.ini$") -> (offset past match=w440:i32)  [unwired: 1 in, 3 out]
          n221 = Format Into String(format string="File %d=\"%s\"\n", initial string=w449, w447, w439) -> (resulting string=w445:string)  [unwired: 1 in, 1 out]
          n222 = String To Path(string=w439) -> (path=w438:path)
          n223 = Greater Or Equal To 0?(x=w440) -> (x >= 0?=w437:bool)
        }
        n224 = Concatenate Strings(w403, "\n" ("string"), w406) -> (w407:string)
        n225 = Unbundle By Name(w410) -> ("BuildPath"=w415:path)
        n226 = local write "Progress"(w407) -> ()
        n227 = Build Path(base path=w415, name or relative path="spec") -> (appended path=w414:path)
        n228 = Write to Text File(file (use dialog)=w414, text=w398, error in=w411) -> (error out=w402:errorcluster)  [unwired: 1 in, 2 out]
        n229 = local read "Output Folder"() -> (w399:path)
        n230 = Build Path(base path=w399, name or relative path="spec_File.txt") -> (appended path=w396:path)
        n231 = Bundle By Name(cluster=w410, "IniFiles"=w386, "SpecFile"=w396) -> (w397:T1)
        n232 = Write to Text File(file (use dialog)=w396, text=w398, error in=w402) -> (error out=w401:errorcluster)  [unwired: 1 in, 2 out]
      }
      frame "Add Package Extra Files" {
        # "Copy extra files"
        n233 = Current VI's Path() -> (path=w500:path)
        n234 = Strip Path(path=w500) -> (stripped path=w498:path)  [unwired: 1 out]
        n235 = property class="App"() -> ("App.Dir"=w492:path)  [unwired: 2 in, 2 out]
        n236 = Build Path(base path=w498, name or relative path="vipm-files") -> (appended path=w475:path)
        n237 = Unbundle By Name(w496) -> ("BuildPath"=w481:path)
        n238 = Build Path(base path=w492, name or relative path="LICENSE") -> (appended path=w490:path)
        n239 = Build Path(base path=w475, name or relative path="icon.bmp") -> (appended path=w495:path)
        n240 = Build Path(base path=w475, name or relative path="PreInstall.vi") -> (appended path=w479:path)
        n241 = Build Path(base path=w475, name or relative path="PostInstall.vi") -> (appended path=w473:path)
        n242 = Build Path(base path=w475, name or relative path="PreUninstall.vi") -> (appended path=w472:path)
        n243 = Build Path(base path=w475, name or relative path="PostUninstall.vi") -> (appended path=w471:path)
        n244 = Copy(8:w494, 9:TRUE ("overwrite (F)"), 10:w481, 11:w495) -> (0:w493:errorcluster)  [unwired: 1 in, 2 out]
        n245 = Copy(8:w493, 10:w481, 11:w490) -> (0:w485:errorcluster)  [unwired: 2 in, 2 out]
        n246 = Copy(8:w485, 9:TRUE ("overwrite (F)"), 10:w481, 11:w479) -> (0:w484:errorcluster)  [unwired: 1 in, 2 out]
        n247 = Copy(8:w484, 9:TRUE ("overwrite (F)"), 10:w481, 11:w473) -> (0:w483:errorcluster)  [unwired: 1 in, 2 out]
        n248 = Copy(8:w483, 9:TRUE ("overwrite (F)"), 10:w481, 11:w472) -> (0:w482:errorcluster)  [unwired: 1 in, 2 out]
        n249 = Copy(8:w482, 9:TRUE ("overwrite (F)"), 10:w481, 11:w471) -> (0:w474:errorcluster)  [unwired: 1 in, 2 out]
        n250 = Build Path(base path=w481, name or relative path="File Group 0") -> (appended path=w488:path)
        n251 = Create Folder(path (use dialog)=w488, error in=w474) -> (error out=w487:errorcluster)  [unwired: 1 in, 2 out]
      }
      frame "Copy Source To LabVIEW Versions" {
        # "Copy source files to all LV version selected"
        n252 = Unbundle By Name(w508) -> ("SourceFiles"=w503:path[], "LvVersion"=w506:path[])
        n253 = local read "LV_Versions"() -> (w507:cluster{"LvVersion":string, "Check":bool}[])
        n254 = property class="App"() -> ("App.Dir"=w502:path)  [unwired: 2 in, 2 out]
        n255 = for {
          tunnel: w507 -> [w519] mode=indexing
          tunnel: w506 -> [w511] mode=indexing
          shift-right: [w514] -> w504
          shift-left: w505 -> [w515]
          tunnel: w503 -> [w513]
          tunnel: w502 -> [w512]
          i -> [w517]
          n256 = Unbundle(w519) -> ("LvVersion"=w510:string, "Check"=w509:bool)
          n257 = Greater Than 0?(x=w517) -> (x > 0?=w516:bool)
          n258 = And(x=w509, y=w516) -> (x .and. y?=w518:bool)
          n259 = case shown="False" w518 {
            tunnel: w515 -> [w520 w530]
            tunnel: [w520 w529] -> w514
            tunnel: w513 -> [_ w533]
            tunnel: w512 -> [_ w532]
            tunnel: w511 -> [_ w531]
            tunnel: w510 -> [_ w523]
            frame False {
            }
            frame True {
              n260 = for {
                N -> [w541]
                tunnel: w533 -> [w554] mode=indexing
                tunnel: w532 -> [w555]
                tunnel: w531 -> [w553]
                shift-right: [w534] -> w529
                shift-left: w530 -> [w550]
                i -> [w542]
                stop <- w534 stop-if-true
                n261 = call <vilib>:"Compare Two Paths.vi"("Path 2"=w554, "Path 1"=w555) -> ("Relative Path from 1 to 2"=w552:path)  [unwired: 6 in, 3 out]
                n262 = Build Path(base path=w553, name or relative path=w552) -> (appended path=w548:path)
                n263 = Divide(x=w542, y=w541) -> (x/y=w540:dbl)
                n264 = Strip Path(path=w548) -> (stripped path=w551:path)  [unwired: 1 out]
                n265 = Multiply(x=w540, y=100.0) -> (x*y=→"Progress":dbl)
                n266 = call <vilib>:"Create Directory Recursive.vi"("error in (no error)"=w550, "directory"=w551) -> ("error out"=w549:errorcluster)  [unwired: 3 in, 2 out]
                n267 = call <vilib>:"Check if File or Folder Exists.vi"("error in (no error)"=w549, "path"=w548) -> ("error out"=w547:errorcluster, "file or folder exists?"=w544:bool, "dup path"=w546:path)  [unwired: 7 in]
                n268 = case shown="True" w544 {
                  tunnel: w547 -> [w556 w560]
                  tunnel: w546 -> [_ w559]
                  tunnel: [w556 w557] -> w545
                  frame False {
                  }
                  frame True {
                    n269 = Set Permissions(7:i16 511 ("permissions"), 8:w560, 11:w559) -> (0:w557:errorcluster)  [unwired: 2 in, 1 out]
                  }
                }
                n270 = Copy(8:w545, 9:TRUE ("overwrite (F)"), 10:w548, 11:w554) -> (0:w535:errorcluster, 3:w536:path)  [unwired: 1 in, 1 out]
                n271 = Set Permissions(7:i16 511 ("permissions"), 8:w535, 11:w536) -> (0:w534:errorcluster)  [unwired: 2 in, 1 out]
              }
              n272 = Format Date/Time String(time format string (%c)="%H:%M:%S") -> (date/time string=w521:string)  [unwired: 2 in]
              n273 = local read "Progress"() -> (w527:string)
              n274 = Format Into String(format string="Copy Files to: %s", initial string=w521, w523) -> (resulting string=w524:string)  [unwired: 1 in, 1 out]
              n275 = Concatenate Strings(w524, "\n" ("string"), w527) -> (w528:string)
              n276 = local write "Progress"(w528) -> ()
            }
          }
        }
      }
      frame "Copy Installer VI to Build Folder" {
        # "Copy and modify Installer VI"
        n277 = Current VI's Path() -> (path=w587:path)
        n278 = Strip Path(path=w587) -> (stripped path=w586:path)  [unwired: 1 out]
        n279 = local read "Output Folder"() -> (w561:path)
        n280 = Strip Path(path=w586) -> (stripped path=w585:path)  [unwired: 1 out]
        n281 = Build Path(base path=w585, name or relative path="Installer") -> (appended path=w583:path)
        n282 = Build Path(base path=w561, name or relative path="Installer.vi") -> (appended path=w562:path)
        n283 = Build Path(base path=w583, name or relative path="OpenGDS_Installer.vi") -> (appended path=w581:path)
        n284 = Open VI Reference(vi path=w581, error in (no error)=w564) -> (vi reference=w580:refnum<vi>, error out=w579:errorcluster)  [unwired: 4 in]
        n285 = invoke class="VI" method="Save.Instrument"(reference=w580, error in=w579, "Path to saved file"=w562) -> (reference out=w576:refnum<vi>, error out=w577:errorcluster)  [unwired: 3 in, 4 out]
        n286 = Bundle By Name(cluster=w588, "InstallerCopy"=w562) -> (w563:T1)
        n287 = call <vilib>:"Traverse for GObjects.vi"("Traverse Target"=TRef_TravTarget."BD", "error in (no error)"=w577, "Class Name"="EnumConstant", "VI Refnum"=w576) -> ("error out"=w572:errorcluster, "References"=w573:refnum<vi>[], "dup VI Refnum"=w568:refnum<vi>)  [unwired: 4 in, 1 out]
        n288 = for {
          tunnel: w573 -> [w599] mode=indexing
          shift-right: [w591] -> w571
          shift-left: w572 -> [w597]
          tunnel: [w590] -> w570 mode=indexing
          w598 = refnum<vi> refnum  # EnumConstant
          n289 = To More Specific Class(target class=w598, reference=w599, error in=w597) -> (specific class reference=w594:refnum<vi>, error out=w596:errorcluster)
          n290 = property class="EnmCnst"(reference=w594, error in=w596) -> (reference out=w593:refnum<vi>, error out=w595:errorcluster, "Typedef?"=w592:T6)
          n291 = case shown="\"typedef\", \"strict typedef\"" w592 {
            tunnel: w595 -> [w601 w605]
            tunnel: w593 -> [w600 w604]
            tunnel: [w601 w603] -> w591
            tunnel: [w600 w602] -> w590
            frame "not a typedef", Default {
            }
            frame "typedef", "strict typedef" {
              n292 = invoke class="EnmCnst" method="Discon Typedef"(reference=w604, error in=w605) -> (reference out=w602:refnum<vi>, error out=w603:errorcluster)  [unwired: 1 in, 1 out]
            }
          }
        }
        n293 = Close Reference(reference=w570, error in (no error)=w571) -> (error out=w569:errorcluster)
        n294 = invoke class="VI" method="Save.Instrument"(reference=w568, error in=w569) -> (reference out=w566:refnum<vi>, error out=w567:errorcluster)  [unwired: 4 in, 4 out]
        n295 = Close Reference(reference=w566, error in (no error)=w567) -> (error out=w565:errorcluster)
      }
      frame "Create Build Process" {
        # "Queue up the state machine"
        n296 = local read "LV_Versions"() -> (w616:cluster{"LvVersion":string, "Check":bool}[])
        n297 = Unbundle By Name(w615) -> ("LvVersion"=w614:path[])
        n298 = for {
          tunnel: w616 -> [w632] mode=indexing
          tunnel: w614 -> [_] mode=indexing
          tunnel: [w622] -> w613 mode=indexing if=w621
          tunnel: [w618] -> w609 mode=indexing
          i -> [w626]
          n299 = Unbundle By Name(w632) -> ("Check"=w627:bool, "LvVersion"=w630:string)
          n300 = Equal To 0?(x=w626) -> (x = 0?=w625:bool)
          n301 = Or(x=w625, y=w627) -> (x .or. y?=w621:bool)
          n302 = Search and Replace String(input string=w630, search string="LabVIEW ", replace string="LV" ("replace string (\"\")")) -> (result string=w618:string)  [unwired: 5 in, 3 out]
          n303 = case shown="False" w625 {
            tunnel: [w634 _] -> w624
            tunnel: w618 -> [w633 _]
            frame False {
              n304 = Format Into String(format string="Mass Compile>>%s\n", w633) -> (resulting string=w634:string)  [unwired: 2 in, 1 out]
            }
            frame True {
            }
          }
          n305 = Format Into String(format string="Copy Files to Package>>%s\nUpdate Spec File>>%s\nCreate Package File>>%s\nCreate ReadMe File>>%s\nZip Installation>>%s\n", w618, w618, w618, w618, w618) -> (resulting string=w623:string)  [unwired: 2 in, 1 out]
          n306 = Format Into String(format string="Update Installer>>%s\n", w618) -> (resulting string=w619:string)  [unwired: 2 in, 1 out]
          n307 = Concatenate Strings(w619, w624, w623) -> (w622:string)
        }
        n308 = Bundle By Name(cluster=w615, "LvVersion"=w609) -> (w610:T1)
        n309 = Build Array (concatenate)(w613, "CleanUpFolder\nUpdateLandingPageLinks\nCopyReleasestoGitHubFolder\nDone") -> (w612:string[])
        n310 = Concatenate Strings(w612) -> (w611:string)
        n311 = Bundle By Name(cluster=w610, "ZipFilesCreated"=path[] []) -> (w607:T1)
      }
      frame "------------------------------------" {
      }
      frame "Update Installer" {
        # "Update Installer"
        n312 = Unbundle By Name(w686) -> ("InstallerCopy"=w684:path, "VersionName"=w647:string)
        n313 = local read "Output Folder"() -> (w683:path)
        n314 = Format Into String(format string="Installer_OpenGDS_%s_%s.vi", w647, w639) -> (resulting string=w678:string)  [unwired: 2 in, 1 out]
        n315 = Build Path(base path=w683, name or relative path=w678) -> (appended path=w682:path)
        n316 = Format Into String(format string="OpenGDS_%s_%s.vip", w647, w639) -> (resulting string=w665:string)  [unwired: 2 in, 1 out]
        n317 = Format Into String(format string="ogds%s", w639) -> (resulting string=w645:string)  [unwired: 2 in, 1 out]
        n318 = Copy(8:w680, 9:TRUE ("overwrite (F)"), 10:w682, 11:w684) -> (0:w677:errorcluster, 3:w662:path)  [unwired: 1 in, 1 out]
        n319 = property class="App"() -> ("App.Dir"=w658:path)  [unwired: 2 in, 2 out]
        n320 = Open VI Reference(vi path=w662, error in (no error)=w677) -> (vi reference=w668:refnum<vi>, error out=w669:errorcluster)  [unwired: 4 in]
        n321 = call <vilib>:"Traverse for GObjects.vi"("Traverse Target"=TRef_TravTarget."BD", "error in (no error)"=w669, "Class Name"="StringConstant", "VI Refnum"=w668) -> ("error out"=w674:errorcluster, "References"=w675:refnum<vi>[], "dup VI Refnum"=w643:refnum<vi>)  [unwired: 4 in, 1 out]
        n322 = Build Path(base path=w658, name or relative path="LICENSE") -> (appended path=w656:path)
        n323 = Format Into String(format string="OpenGDS %s", w647) -> (resulting string=w648:string)  [unwired: 2 in, 1 out]
        n324 = for {
          tunnel: w675 -> [w717] mode=indexing
          shift-right: [w709] -> w673
          shift-left: w674 -> [w715]
          tunnel: [w708] -> w672 mode=indexing
          tunnel: w665 -> [w707]
          tunnel: w648 -> [w706]
          tunnel: w645 -> [w705]
          w716 = refnum<vi> refnum  # StringConstant
          n325 = To More Specific Class(target class=w716, reference=w717, error in=w715) -> (specific class reference=w712:refnum<vi>, error out=w714:errorcluster)
          n326 = property class="StrCnst"(reference=w712, error in=w714) -> (reference out=w711:refnum<vi>, error out=w713:errorcluster, "Label.Text"=w710:string)
          n327 = case shown="\"TempFolderName\"" w710 {
            tunnel: w713 -> [w719 w724 w729 w734]
            tunnel: w711 -> [w718 w723 w728 w733]
            tunnel: [w719 w722 w727 w732] -> w709
            tunnel: [w718 w721 w726 w731] -> w708
            tunnel: w707 -> [_ w720 _ _]
            tunnel: w706 -> [_ _ _ w730]
            tunnel: w705 -> [_ _ w725 _]
            frame Default {
            }
            frame "VIP-File" {
              n328 = property class="StrCnst"(reference=w723, error in=w724, "Value"=w720) -> (reference out=w721:refnum<vi>, error out=w722:errorcluster)
            }
            frame "TempFolderName" {
              n329 = property class="StrCnst"(reference=w728, error in=w729, "Value"=w725) -> (reference out=w726:refnum<vi>, error out=w727:errorcluster)
            }
            frame "Version" {
              n330 = property class="StrCnst"(reference=w733, error in=w734, "Value"=w730) -> (reference out=w731:refnum<vi>, error out=w732:errorcluster)
            }
          }
        }
        n331 = Read from Text File(file (use dialog)=w656) -> (text=w655:string)  [unwired: 3 in, 3 out]
        n332 = Bundle By Name(cluster=w686, "InstallerFile"=w662) -> (w663:T1)
        n333 = Close Reference(reference=w672, error in (no error)=w673) -> (error out=w660:errorcluster)
        n334 = call <vilib>:"Traverse for GObjects.vi"("Traverse Target"=TRef_TravTarget."FP", "error in (no error)"=w660, "Class Name"="String", "VI Refnum"=w643) -> ("error out"=w650:errorcluster, "References"=w651:refnum<vi>[])  [unwired: 4 in, 2 out]
        n335 = for {
          tunnel: w651 -> [w697] mode=indexing
          shift-right: [w689] -> w654
          shift-left: w650 -> [w695]
          tunnel: [w688] -> w653 mode=indexing
          tunnel: w655 -> [w687]
          w696 = refnum<vi> refnum  # String
          n336 = To More Specific Class(target class=w696, reference=w697, error in=w695) -> (specific class reference=w692:refnum<vi>, error out=w694:errorcluster)
          n337 = property class="Str"(reference=w692, error in=w694) -> (reference out=w691:refnum<vi>, error out=w693:errorcluster, "Label.Text"=w690:string)
          n338 = case shown="\"Lic\"" w690 {
            tunnel: w693 -> [w699 w704]
            tunnel: w691 -> [w698 w703]
            tunnel: [w699 w702] -> w689
            tunnel: [w698 w700] -> w688
            tunnel: w687 -> [_ w701]
            frame Default {
            }
            frame "Lic" {
              n339 = property class="Str"(reference=w703, error in=w704, "Value"=w701) -> (reference out=w700:refnum<vi>, error out=w702:errorcluster)
            }
          }
        }
        n340 = Close Reference(reference=w653, error in (no error)=w654) -> (error out=w652:errorcluster)
        n341 = invoke class="VI" method="Default Vals.Make Curr Default"(reference=w643, error in=w652) -> (error out=w641:errorcluster)  [unwired: 1 in, 2 out]
        n342 = property class="VI"(reference=w643, error in=w641, "Exec.RunOnOpen"=TRUE ("Execution:Run When Opened")) -> (reference out=w642:refnum<vi>, error out=w644:errorcluster)
        n343 = invoke class="VI" method="Save.Instrument"(reference=w642, error in=w644) -> (reference out=w670:refnum<vi>, error out=w671:errorcluster)  [unwired: 4 in, 4 out]
        n344 = Close Reference(reference=w670, error in (no error)=w671) -> (error out=w664:errorcluster)
      }
      frame "Mass Compile" {
        # "\"C:\\Program Files\\National Instruments\\LabVIEW 2013\\LabVIEW.exe\" \"C:\\Program Files (x86)\\National Instruments\\LabVIEW 2012\\Open_GDS_Tools\\Build_Release\\BuildRelease_SubVIs\\BuildRelease_RecompileOpenGDS.vi\" -- \"2120\" \"C:\\...\\spec\""
        # "Mass Compile"
        n345 = Unbundle By Name(w770) -> ("SourceFiles"=w760:path[], "LvVersion"=w779:path[], "LvVersion"=w781:string[])
        n346 = Unbundle By Name(w770) -> ("BuildPath"=w748:path, "SpecFile"=w769:path, "InstallerFile"=w747:path, "LogFolder"=w746:path, "IniFiles"=w764:path[])
        n347 = vi-ref "BuildRelease_RecompileOpenGDS_RemoveDebugFlag.vi"() -> (w739:refnum<vi>)
        n348 = vi-ref "BuildRelease_RecompileOpenGDS.vi"() -> (w775:refnum<vi>)
        n349 = property class="VI"(reference=w775, error in=w735) -> (error out=w772:errorcluster, "Path"=w773:path)  [unwired: 1 out]
        n350 = property class="VI"(reference=w739, error in=w735) -> (error out=w742:errorcluster, "Path"=w741:path)  [unwired: 1 out]
        n351 = Search 1D Array(1D array=w781, element=w780) -> (index of element=w778:i32)  [unwired: 1 in]
        n352 = local read "Output Folder"() -> (w768:path)
        n353 = Set Permissions(7:i16 365 ("permissions"), 8:w772, 11:w773) -> (0:w737:errorcluster, 3:w771:path)  [unwired: 2 in]
        n354 = Set Permissions(7:i16 365 ("permissions"), 8:w742, 11:w741) -> (0:w738:errorcluster)  [unwired: 2 in, 1 out]
        n355 = Index Array(array=w779, index=w778) -> (element=w744:path)
        n356 = Merge Errors(w737, w738) -> (w736:errorcluster)
        n357 = Build Path(base path=w768, name or relative path="TempFolder") -> (appended path=w766:path)
        n358 = for {
          shift-right: [w807] -> w750
          shift-left: w736 -> [w808]
          tunnel: w764 -> [w803] mode=indexing
          tunnel: w766 -> [w806]
          tunnel: [w804] -> w765 mode=indexing
          tunnel: w744 -> [w802]
          tunnel: [w801] -> w743 mode=indexing
          # "Remove ini files\nbefore starting LV"
          n359 = Build Path(base path=w802, name or relative path=w803) -> (appended path=w801:path)
          n360 = Move(source path=w801, error in=w808, 9:TRUE ("overwrite (F)"), 10:w806) -> (error out=w807:errorcluster, 3:w804:path)  [unwired: 1 in, 1 out]
        }
        n361 = Current VI's Path() -> (path=w752:path)
        n362 = Strip Path(path=w752) -> (stripped path=w745:path)  [unwired: 1 out]
        n363 = Format Into String(format string="\"%s\\\\LabVIEW.exe\" \"%s\" -- \"%s\" \"%s\" \"%s\" \"%s\"", w744, w771, w748, w769, w747, w746) -> (resulting string=w776:string)  [unwired: 2 in, 1 out]
        n364 = Build Path(base path=w745, name or relative path="vipm-files") -> (appended path=w757:path)
        n365 = for {
          tunnel: w760 -> [w793] mode=indexing
          tunnel: w744 -> [w795]
          tunnel: [w794] -> w759 mode=indexing
          n366 = Path To String(path=w793) -> (string=w792:string)
          n367 = Match Pattern(string=w792, regular expression="LabVIEW [0-9]+\\\\") -> (after substring=w790:string)  [unwired: 1 in, 3 out]
          n368 = Build Path(base path=w795, name or relative path=w790) -> (appended path=w794:path)
        }
        n369 = Build Array("PreInstall.vi" ("name or relative path"), "PostInstall.vi" ("name or relative path"), "PreUninstall.vi" ("name or relative path"), "PostUninstall.vi" ("name or relative path")) -> (w758:string[])
        n370 = for {
          tunnel: w757 -> [w789]
          tunnel: w758 -> [w788] mode=indexing
          shift-right: [w785] -> w749
          shift-left: w750 -> [w786]
          tunnel: w748 -> [w783]
          n371 = Build Path(base path=w789, name or relative path=w788) -> (appended path=w787:path)
          n372 = Copy(8:w786, 9:TRUE ("overwrite (F)"), 10:w783, 11:w787) -> (0:w785:errorcluster)  [unwired: 1 in, 2 out]
        }
        n373 = call <vilib>:"System Exec.vi"("error in (no error)"=w749, "command line"=w776) -> ("error out"=w763:errorcluster)  [unwired: 6 in, 3 out]
        n374 = Bundle By Name(cluster=w770, "SourceFiles"=w759) -> (w761:T1)
        n375 = for {
          shift-right: [w799] -> w762
          shift-left: w763 -> [w800]
          tunnel: w765 -> [w798] mode=indexing
          tunnel: w743 -> [w797] mode=indexing
          # "Restore ini files"
          n376 = Move(source path=w798, error in=w800, 9:TRUE ("overwrite (F)"), 10:w797) -> (error out=w799:errorcluster)  [unwired: 1 in, 2 out]
        }
      }
      frame "Update Spec File" {
        (unwired) "%sExclusive_LabVIEW_Version=\">=%s\"%s" ("format string")
        (unwired) "%sExclusive_LabVIEW_Version=\">=%s.0\"%s" ("format string")
        # "\"C:\\Program Files\\National Instruments\\LabVIEW 2013\\LabVIEW.exe\" \"C:\\Program Files (x86)\\National Instruments\\LabVIEW 2012\\Open_GDS_Tools\\Build_Release\\BuildRelease_SubVIs\\BuildRelease_RecompileOpenGDS.vi\" -- \"2120\" \"C:\\...\\spec\""
        # "Mass Compile"
        n377 = Unbundle By Name(w825) -> ("LvVersion"=w827:path[], "LvVersion"=w829:string[])  [unwired: 1 out]
        n378 = Unbundle By Name(w825) -> ("BuildPath"=w823:path)
        n379 = Search 1D Array(1D array=w829, element=w828) -> (index of element=w826:i32)  [unwired: 1 in]
        n380 = Build Path(base path=w823, name or relative path="spec") -> (appended path=w810:path)
        n381 = Index Array(array=w827, index=w826) -> (element=w814:path)
        n382 = Path To String(path=w814) -> (string=w813:string)
        n383 = Read from Text File(file (use dialog)=w810, error in=w824) -> (text=w820:string, error out=w821:errorcluster)  [unwired: 2 in, 2 out]
        n384 = Match Pattern(string=w813, regular expression="[0-9][0-9]$") -> (match substring=w811:string)  [unwired: 1 in, 3 out]
        n385 = Match Pattern(string=w820, regular expression="Exclusive_LabVIEW_Version=\"[~\"]+\"") -> (before substring=w818:string, after substring=w817:string)  [unwired: 1 in, 2 out]
        n386 = Format Into String(format string="%sExclusive_LabVIEW_Version=\">=%s.0\"%s", w818, w811, w817) -> (resulting string=w816:string)  [unwired: 2 in, 1 out]
        n387 = Write to Text File(file (use dialog)=w810, text=w816, error in=w821) -> (error out=w809:errorcluster)  [unwired: 1 in, 2 out]
      }
      frame "Copy Files to Package" {
        # "Copy Source files"
        n388 = Unbundle By Name(w832) -> ("BuildPath"=w845:path, "SourceFiles"=w843:path[])
        n389 = Unbundle By Name(w832) -> ("LvVersion"=w837:path[], "LvVersion"=w839:string[])
        n390 = Search 1D Array(1D array=w839, element=w836) -> (index of element=w838:i32)  [unwired: 1 in]
        n391 = Index Array(array=w837, index=w838) -> (element=w835:path)
        n392 = Build Path(base path=w845, name or relative path="File Group 0") -> (appended path=w834:path)
        n393 = call <vilib>:"Create Directory Recursive.vi"("directory"=w834) -> ("directory copy"=w833:path)  [unwired: 4 in, 2 out]
        n394 = for {
          N -> [w863]
          tunnel: w843 -> [w854] mode=indexing
          tunnel: w835 -> [w868]
          shift-right: [w856] -> w841
          shift-left: w842 -> [w867]
          tunnel: w833 -> [w865]
          tunnel: [w855] -> w831 mode=indexing if=w857
          i -> [w864]
          stop <- w856 stop-if-true
          n395 = Increment(x=w864) -> (x+1=w846:i32)
          n396 = call <vilib>:"Compare Two Paths.vi"("error in (no error)"=w867, "Path 2"=w854, "Path 1"=w868) -> ("error out"=w850:errorcluster, "Relative Path from 1 to 2"=w866:path)  [unwired: 5 in, 2 out]
          n397 = Divide(x=w846, y=w863) -> (x/y=w847:dbl)
          n398 = Build Path(base path=w865, name or relative path=w866) -> (appended path=w851:path)
          n399 = Multiply(x=w847, y=100) -> (x*y=w861:dbl)
          n400 = Strip Path(path=w851) -> (stripped path=w848:path)  [unwired: 1 out]
          n401 = local write "Progress"(w861) -> ()
          n402 = call <vilib>:"Create Directory Recursive.vi"("error in (no error)"=w850, "directory"=w848) -> ("error out"=w849:errorcluster)  [unwired: 3 in, 2 out]
          n403 = File/Directory Info(path=w854, error in=w849) -> (directory=w852:bool, error out=w853:errorcluster)  [unwired: 5 out]
          n404 = case shown="False" w852 {
            tunnel: [w875 w876] -> w856
            tunnel: w851 -> [w872 _]
            tunnel: [w871 _] -> w855
            tunnel: w854 -> [w870 _]
            tunnel: w853 -> [w869 w876]
            frame False {
              n405 = Set Permissions(7:i16 511 ("permissions"), 11:w872) -> (3:w871:path)  [unwired: 3 in, 1 out]
              n406 = Copy(8:w869, 9:TRUE ("overwrite (F)"), 10:w871, 11:w870) -> (0:w875:errorcluster)  [unwired: 1 in, 2 out]
            }
            frame True {
            }
          }
          n407 = Strip Path(path=w855) -> (name=w860:string)  [unwired: 1 out]
          n408 = Match Pattern(string=w860, regular expression="^GOOP_[A-Za-z]+.ini$") -> (offset past match=w858:i32)  [unwired: 1 in, 3 out]
          n409 = Greater Or Equal To 0?(x=w858) -> (x >= 0?=w857:bool)
        }
      }
      frame "Create Package File" {
        # "Copy extra files"
        n410 = Unbundle By Name(w896) -> ("BuildPath"=w880:path, "VersionName"=w879:string)
        n411 = local read "Output Folder"() -> (w887:path)
        n412 = call <vilib>:"Recursive File List.vi"("error in (no error)"=w895, "Folder Path"=w880) -> ("error out"=w888:errorcluster, "All Files in Dir"=w889:path[])  [unwired: 5 in, 3 out]
        n413 = Format Into String(format string="OpenGDS_%s_%s.vip", w879, w885) -> (resulting string=w884:string)  [unwired: 2 in, 1 out]
        n414 = Build Path(base path=w887, name or relative path=w884) -> (appended path=w877:path)
        n415 = Bundle By Name(cluster=w896, "VIP-File"=w877) -> (w878:T1)
        n416 = Delete(path (use dialog)=w877) -> (deleted path=w882:path)  [unwired: 4 in, 2 out]
        n417 = call <vilib>:"New Zip File.vi"("error in (no error)"=w888, "confirm overwrite? (F)"=TRUE, "target"=w882) -> ("error out"=w892:errorcluster, "zip file out"=w893:i64)  [unwired: 2 in, 1 out]
        n418 = for {
          N -> [w900]
          tunnel: w889 -> [w905] mode=indexing
          shift-right: [w907] -> w890
          shift-left: w893 -> [w909]
          shift-right: [w899] -> w891
          shift-left: w892 -> [w908]
          tunnel: w880 -> [w906]
          i -> [w901]
          stop <- w899 stop-if-true
          n419 = Increment(x=w901) -> (x+1=w897:i32)
          n420 = Divide(x=w897, y=w900) -> (x/y=w898:dbl)
          n421 = call <vilib>:"Compare Two Paths.vi"("Path 2"=w905, "Path 1"=w906) -> ("Relative Path from 1 to 2"=w904:path)  [unwired: 6 in, 3 out]
          n422 = Multiply(x=w898, y=100) -> (x*y=w902:dbl)
          n423 = call <vilib>:"Add File to Zip.vi"("error in (no error)"=w908, "destination path in zip"=w904, "source file path"=w905, "zip file in"=w909) -> ("error out"=w899:errorcluster, "zip file out"=w907:i64)  [unwired: 6 in]
          n424 = local write "Progress"(w902) -> ()
        }
        n425 = call <vilib>:"Close Zip File.vi"("error in (no error)"=w891, "zip file in"=w890) -> ("error out"=w883:errorcluster)  [unwired: 5 in]
      }
      frame "Create ReadMe File" {
        # "Update Installer"
        n426 = Unbundle By Name(w924) -> ("InstallerFile"=w911:path, "VersionName"=w913:string)
        n427 = local read "Output Folder"() -> (w922:path)
        n428 = Strip Path(path=w911) -> (name=w910:string)  [unwired: 1 out]
        n429 = Format Into String(format string="ReadMe_OpenGDS_%s_%s.txt", w913, w912) -> (resulting string=w920:string)  [unwired: 2 in, 1 out]
        n430 = Build Path(base path=w922, name or relative path=w920) -> (appended path=w918:path)
        n431 = Format Into String(format string="Welcome to OpenGDS\nThis is the release: %s, build for: %s\nTo install this version use either, VIPM or the installer VI (%s)." ("text"), w913, w912, w910) -> (resulting string=w914:string)  [unwired: 2 in, 1 out]
        n432 = Bundle By Name(cluster=w924, "ReadMeFile"=w918) -> (w919:T1)
        n433 = Write to Text File(file (use dialog)=w918, text=w914, error in=w917) -> (error out=w916:errorcluster)  [unwired: 1 in, 2 out]
      }
      frame "Zip Installation" {
        # "Zip Installtion"
        n434 = Build Path(base path=w928, name or relative path=path "releases") -> (appended path=w926:path)
        n435 = Unbundle By Name(w929) -> ("VIP-File"=w939:path, "ReadMeFile"=w938:path, "InstallerFile"=w937:path)
        n436 = Unbundle By Name(w929) -> ("VersionName"=w933:string)
        n437 = call <vilib>:"Check if File or Folder Exists.vi"("path"=w926) -> ()  [unwired: 8 in, 3 out]
        n438 = local read "Output Folder"() -> (w934:path)
        n439 = Format Into String(format string="OpenGDS_%s_%s.zip", w933, w944) -> (resulting string=w943:string)  [unwired: 2 in, 1 out]
        n440 = Build Array(w939, w938, w937) -> (w935:path[])
        n441 = Build Path(base path=w934, name or relative path=w943) -> (appended path=w941:path)
        n442 = Unbundle By Name(w929) -> ("ZipFilesCreated"=w931:path[])
        n443 = Delete(path (use dialog)=w941) -> (deleted path=w925:path)  [unwired: 4 in, 2 out]
        n444 = call <vilib>:"New Zip File.vi"("error in (no error)"=w936, "confirm overwrite? (F)"=TRUE, "target"=w925) -> ("error out"=w948:errorcluster, "zip file out"=w949:i64)  [unwired: 2 in, 1 out]
        n445 = for {
          N -> [w954]
          tunnel: w935 -> [w959] mode=indexing
          shift-right: [w961] -> w946
          shift-left: w949 -> [w963]
          shift-right: [w953] -> w947
          shift-left: w948 -> [w962]
          tunnel: w934 -> [w960]
          i -> [w955]
          stop <- w953 stop-if-true
          n446 = Increment(x=w955) -> (x+1=w951:i32)
          n447 = Divide(x=w951, y=w954) -> (x/y=w952:dbl)
          n448 = call <vilib>:"Compare Two Paths.vi"("Path 2"=w959, "Path 1"=w960) -> ("Relative Path from 1 to 2"=w958:path)  [unwired: 6 in, 3 out]
          n449 = Multiply(x=w952, y=100) -> (x*y=w956:dbl)
          n450 = call <vilib>:"Add File to Zip.vi"("error in (no error)"=w962, "destination path in zip"=w958, "source file path"=w959, "zip file in"=w963) -> ("error out"=w953:errorcluster, "zip file out"=w961:i64)  [unwired: 6 in]
          n451 = local write "Progress"(w956) -> ()
        }
        n452 = Build Array (concatenate)(w931, w925) -> (w930:path[])
        n453 = Bundle By Name(cluster=w929, "ZipFilesCreated"=w930) -> (w932:T1)
        n454 = call <vilib>:"Close Zip File.vi"("error in (no error)"=w947, "zip file in"=w946) -> ("error out"=w942:errorcluster)  [unwired: 5 in]
      }
      frame "CleanUpFolder" {
        n455 = local read "Output Folder"() -> (w968:path)
        n456 = Build Path(base path=w968, name or relative path="TempFolder") -> (appended path=w972:path)
        n457 = List Folder(path=w968, pattern="*.txt" ("name or relative path")) -> (path out=w966:path, filenames=w967:string[])  [unwired: 2 in, 2 out]
        n458 = List Folder(path=w968, pattern="*.vi" ("name or relative path")) -> (path out=w965:path, filenames=w964:string[])  [unwired: 2 in, 2 out]
        n459 = for {
          tunnel: w967 -> [w982] mode=indexing
          tunnel: w966 -> [w981]
          n460 = Build Path(base path=w981, name or relative path=w982) -> (appended path=w980:path)
          n461 = Delete(path (use dialog)=w980) -> ()  [unwired: 4 in, 3 out]
        }
        n462 = for {
          tunnel: w964 -> [w979] mode=indexing
          tunnel: w965 -> [w978]
          n463 = Build Path(base path=w978, name or relative path=w979) -> (appended path=w977:path)
          n464 = Delete(path (use dialog)=w977) -> ()  [unwired: 4 in, 3 out]
        }
        n465 = Delete(path (use dialog)=w972, entire hierarchy (F)=TRUE) -> ()  [unwired: 3 in, 3 out]
      }
      frame "UpdateLandingPageLinks" {
        n466 = Build Path(base path=w988, name or relative path=path "index.html") -> (appended path=w986:path)
        n467 = call <vilib>:"Check if File or Folder Exists.vi"("path"=w986) -> ("file or folder exists?"=w985:bool, "dup path"=w984:path)  [unwired: 8 in, 1 out]
        n468 = case shown="True" w985 {
          tunnel: w984 -> [_ w991]
          tunnel: w983 -> [_ w999]
          frame False {
          }
          frame True {
            n469 = Read from Text File(file (use dialog)=w991) -> (text=w1004:string)  [unwired: 3 in, 3 out]
            n470 = Unbundle By Name(w999) -> ("ZipFilesCreated"=w998:path[])
            n471 = Match Pattern(string=w1004, regular expression="id=\"untestedversions\"") -> (offset past match=w1002:i32)  [unwired: 1 in, 3 out]
            n472 = Match Pattern(string=w1004, regular expression="<a", offset (0)=w1002) -> (before substring=w996:string, after substring=w1001:string)  [unwired: 2 out]
            n473 = Match Pattern(string=w1001, regular expression="</div>") -> (match substring=w994:string, after substring=w993:string)  [unwired: 1 in, 2 out]
            n474 = for {
              tunnel: w998 -> [w1009] mode=indexing
              tunnel: "<a href=\"https://opengds.github.io/releases/%1$s\">%1$s</a><BR>\n" ("regular expression") -> [w1008]
              tunnel: [w1006] -> w995 mode=indexing
              n475 = Strip Path(path=w1009) -> (name=w1007:string)  [unwired: 1 out]
              n476 = Format Into String(format string=w1008, w1007) -> (resulting string=w1006:string)  [unwired: 2 in, 1 out]
            }
            n477 = Concatenate Strings(w996, w995, w994, w993) -> (w992:string)
            n478 = Write to Text File(file (use dialog)=w991, text=w992) -> ()  [unwired: 2 in, 3 out]
          }
        }
      }
      frame "CopyReleasestoGitHubFolder" {
        n479 = Build Path(base path=w1012, name or relative path=path "releases") -> (appended path=w1015:path)
        n480 = call <vilib>:"Check if File or Folder Exists.vi"("path"=w1015) -> ("file or folder exists?"=w1014:bool, "dup path"=w1013:path)  [unwired: 8 in, 1 out]
        n481 = case shown="True" w1014 {
          tunnel: w1013 -> [_ w1018]
          tunnel: w1010 -> [_ w1020]
          frame False {
          }
          frame True {
            n482 = Unbundle By Name(w1020) -> ("ZipFilesCreated"=w1019:path[])
            n483 = for {
              tunnel: w1019 -> [w1022] mode=indexing
              tunnel: w1018 -> [w1021]
              n484 = Copy(9:TRUE ("overwrite (F)"), 10:w1021, 11:w1022) -> ()  [unwired: 2 in, 3 out]
            }
          }
        }
      }
    }
    n485 = local write "Progress"(w18) -> ()
  }
